vi "Orca Flash Capture Manager.vi"(7 "Calling VI Ref":refnum<vi>) -> ()   [LabVIEW 2016]
uses:
  Orca Flash Capture Manager Controls/Orca Flash Capture Switch Line Scan Modes.ctl
  Orca Flash Capture Manager Controls/Orca Flash Capture Line Scan Settings.ctl
  Orca Flash Capture Manager Controls/Orca Flash Switch Cycles Steps.ctl
  <vilib>/Utility/miscctls.llb/LVPointTypeDef.ctl
  Orca Flash Capture Manager Controls/Orca Flash Capture Notifier Type.ctl
  Orca Flash Capture Manager Controls/Orca Flash Capture Actions.ctl
  <vilib>/vision/Image Controls.llb/IMAQ Image.ctl
  Hardware Configuration/Hardware Configuration Controls/Device Type.ctl
  Orca Flash Capture Manager Controls/Orca Flash Capture Line Scan Filter Settings.ctl
  Tools/Log File/Log File Type Defs/Log File Actions.ctl
  Hardware Configuration/Hardware Configuration Controls/Device Function.ctl
  Device Library/Cameras/Hamamatsu/Orca Flash/Orca Flash Controls/Orca Flash Actions.ctl
  Device Library/Cameras/Hamamatsu/Orca Flash/Orca Flash Controls/Orca Flash Parameters.ctl
  Device Library/Cameras/Hamamatsu/Orca Flash/Orca Flash Controls/Orca Flash Parameter List.ctl
  Device Library/Cameras/Hamamatsu/Orca Flash/Orca Flash Controls/Orca Flash ROI.ctl
  Orca Flash Capture Manager Controls/Orca Flash Capture Cycle Step Count.ctl
  <vilib>/Utility/error.llb/whitespace.ctl
  Device Manager/Common Device Queue/Common Device Controls/Common Device Actions.ctl
  Device Library/SMTP Email Alerts/SMTP Email Alerts Type Defs/SMTP Email Alerts Actions.ctl
  Device Library/DAQmx/AO Single Channel Triggered Ramp/AO SCTR Type Defs/AO SCTR Actions.ctl
  Wide Field Drift Correction/WFDC Controls/WFDC External Sync.ctl
  Wide Field Drift Correction/WFDC Controls/WFDC Cycle Pause.ctl
  Wide Field Drift Correction/WFDC Controls/WFDC Status.ctl
  Device Library/Stages/Stages Controls/Stage Actions.ctl
  Laser Control/Laser Power Control/Laser Power Control Type Defs/Laser Power Ctrl Messenger Actions.ctl
  Device Library/Cameras/Camera Controls/Camera IMAQ Key Info.ctl
  <vilib>/Utility/file.llb/Read Delimited Spreadsheet (DBL).vi
  shell32.dll
panel:
  in  "Main Tab":T1(tab)
  in  "Scan Mode":T2=enum."Cycles Then Steps"
  out "Frame":u32(slide) scale=0.0..20.0
  out "Cycle":sgl(slide) scale=0.0..1.0
  in  "Base Save Path":path
  in  "Capture":bool
  in  "Live Preview":bool
  out "Z Step":sgl(slide) scale=0.0..1.0
  in  "File Name":string="Test Image"
  in  "Preview Exposure Time (s)":dbl=0.1 caption="Frame Rate (Hz)"
  in  "Capture Exposure Time (s)":dbl=0.1 caption="Frame Rate (Hz)"
  in  "No. of Frames":u32=1 min=1
  in  "No. of Cycles":u16=1 min=1
  in  "No. of Z Steps":u16=1 min=1
  in  "Z Step Size (µm)":dbl min=-10.0 max=10.0
  out "Current Cycle":u16
  out "Current Step":u16
  out "Current Frame":u32
  in  "Auto Update Subfolder":bool=TRUE
  in  "Subfolder Name":string="Area"
  in  "Two Color Calibration":bool
  in  "Current Filter":i32(ring) items=["Default"]
  in  "Save As Preset":bool
  in  "Line Scan Active":bool
  in  "Number of Lines":u32=8 min=1 max=200 step=1
  in  "Line Scan Mode":T3
  in  "Line Scanning Presets":u16(ring) items=["04 FPS", "08 FPS Clean", "08 FPS", "40 FPS"]
  in  "Line Scan Settings":T4
  in  "Line Scan Offset Active":bool
  in  "Line Scan Offset (V)":dbl
  in  "Collect Metadata":bool
  in  "Edit Metadata":bool
  in  "Camera Settings":bool
  in  "Quadrants On/Off":bool
  in  "Email Alerts":bool
  in  "Email Address":string
  in  "Auto Laser Off Time (min)":u16=30
  in  "Quit":bool
  # "Live Preview"
  # "Capture"
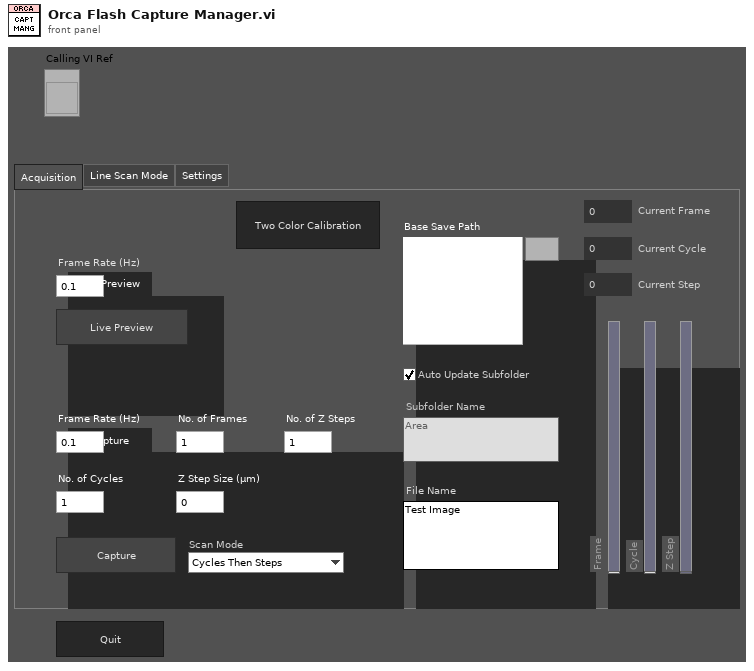
[diagram p1: front panel]
types:
  T1 = enum32{"Acquisition", "Line Scan Mode", "Settings"}
  T2 = typedef "Orca Flash Switch Cycles Steps.ctl" = enum16{"Steps Then Cycles", "Cycles Then Steps"}
  T3 = typedef "Orca Flash Capture Switch Line Scan Modes.ctl" = enum32{"Automatic", "Use Presets", "Manual"}
  T4 = typedef "Orca Flash Capture Line Scan Settings.ctl" = cluster{"Interline Interval":dbl, "Offset (V)":dbl, "Amplitude (V)":dbl, "Samples Per Channel":dbl, "Delay (ms)":dbl}
  T5 = typedef "Log File Actions.ctl" = enum16{"Open File", "Write"}
  T6 = typedef "IMAQ Image.ctl" = refnum<image>
  T7 = cluster{"Image Ref":T6, "Cycle Number":u16, "Camera Running?":bool, "Capture?":bool}
  T8 = typedef "Orca Flash Capture Line Scan Filter Settings.ctl" = cluster{"Filter Name":string, "Offset (V)":dbl}[]
  T9 = enum8{"Enabled", "Disabled", "Disabled and Grayed Out"}
  T10 = typedef "Device Type.ctl" = enum16{"AOTF", "Camera", "Deformable Mirror", "Laser", "Shutter", "Stage", "Waveform", "FPGA", "Email", "Filter Wheel"}
  T11 = typedef "Orca Flash Capture Notifier Type.ctl" = cluster{"Actions":T12, "Running?":bool, "Preview Exposure (s)":dbl, "Capture Exposure (s)":dbl, "Cycles":u16, "Frames":u32, "No. of Z Steps":u16, "Z Step Size (µm)":dbl, "Base Path":path, "Init Z Position (µm)":dbl, "Lasers Lines":string[], "Save Path":path, "Line Scan?":bool, "Line Scan Mode":T3, "Collect Metadata?":bool}
  T12 = typedef "Orca Flash Capture Actions.ctl" = enum16{"Idle", "Live Preview", "Capture", "Check File Name", "Laser On", "Laser Off", "Open Shutters", "Close Shutters", "Set Exposure Time", "Start Acquisition", "Update SubFolder", "Write Metadata", "Setup", "Camera", "Switch", "Step", "Cycle", "External Cycle Sync", "Abort", "Quit"}
  T13 = enum16{"Always On", "Always Off", "Off While Running"}
  T14 = typedef "LVPointTypeDef.ctl" = cluster{"Horizontal":i16, "Vertical":i16}
  T15 = typedef "Image Type" = u32
  T16 = typedef "Device Function.ctl" = enum16{"Primary", "Secondary", "Overview", "Wide Field Drift Correction", "642 nm Excitation", "560 nm Excitation", "940 nm Excitation", "546 nm Excitation", "488 nm Excitation", "405 nm Excitation", "Objective Drift Correction", "4Pi Objective Lock", "Objective XY", "Objective Z", "Sample XY", "Sample Coarse Z", "Sample Z", "4Pi Lower", "4Pi Upper", "Mojo", "Adj Cavity", "Line Scanning", "Alert"}
  T17 = typedef "Orca Flash ROI.ctl" = cluster{"H Offset":i32, "V Offset":i32, "H Width":i32, "V Width":i32}
  T18 = typedef "Orca Flash Parameters.ctl" = cluster{"Value":dbl, "Parameter":T19}
  T19 = typedef "Orca Flash Parameter List.ctl" = u32
  T20 = typedef "Orca Flash Actions.ctl" = enum16{"IDLE", "PREVIEW", "RECORD", "Record Settings", "SETPARAM", "GETPARAM", "SETROI", "GETROI", "PROGRESSIVE MODE", "AREA MODE", "STATUS", "QUIT"}
  T21 = typedef "Orca Flash Capture Cycle Step Count.ctl" = cluster{"Scan Mode":T2, "Current Step":u16, "Current Cycle":u16, "Num of Steps":u16, "Num of Cycles":u16}
  T22 = typedef "WFDC Status.ctl" = enum16{"Idle", "Busy", "DC Active", "Error"}
  T23 = typedef "WFDC External Sync.ctl" = cluster{"Cycle Sync":T24, "Z Offset":dbl, "WFDC Status":T22}
  T24 = typedef "WFDC Cycle Pause.ctl" = enum16{"Pause Requested", "Paused", "Resume Requested", "Resumed"}
  T25 = typedef "SMTP Email Alerts Actions.ctl" = enum16{"Set Recipient", "Send Message", "Quit"}
  T26 = typedef "Stage Actions.ctl" = enum16{"Get Position", "MVR", "MOVE", "HALT", "ONTARGET", "ERROR", "REFERENCE", "INIT", "VELOCITY", "STATUS", "EXIT", "HOME", "ZEROPOS", "NANOPOS", "ANALOG", "QUIT"}
  T27 = typedef "Laser Power Ctrl Messenger Actions.ctl" = enum16{"All Active On", "All Off", "Adjust Power", "Line On/Off", "Get Status"}
  T28 = typedef "AO SCTR Actions.ctl" = enum16{"Stop at Offset", "Update and Run", "Quit"}
  T29 = typedef "Camera IMAQ Key Info.ctl" = cluster{"Frame":u32, "Sensor Height":i32, "Sensor Width":i32, "ROI Height":i32, "ROI Width":i32, "ROI Enable?":bool, "Bit per Pixel":u8}
  T30 = typedef "Common Device Actions.ctl" = enum16{"Specific Action", "Open Front Panel", "Close Front Panel", "Quit", "Quit All"}
  T31 = enum32{"Invalid", "Standard", "Closed", "Hidden", "Minimized", "Maximized"}
  T32 = typedef "whitespace.ctl" = u16
  T33 = typedef "LVRectTypeDef.ctl" = cluster{"Left":i16, "Top":i16, "Right":i16, "Bottom":i16}
  T34 = typedef "LVBoundsTypeDef.ctl" = cluster{"Width":u32, "Height":u32}
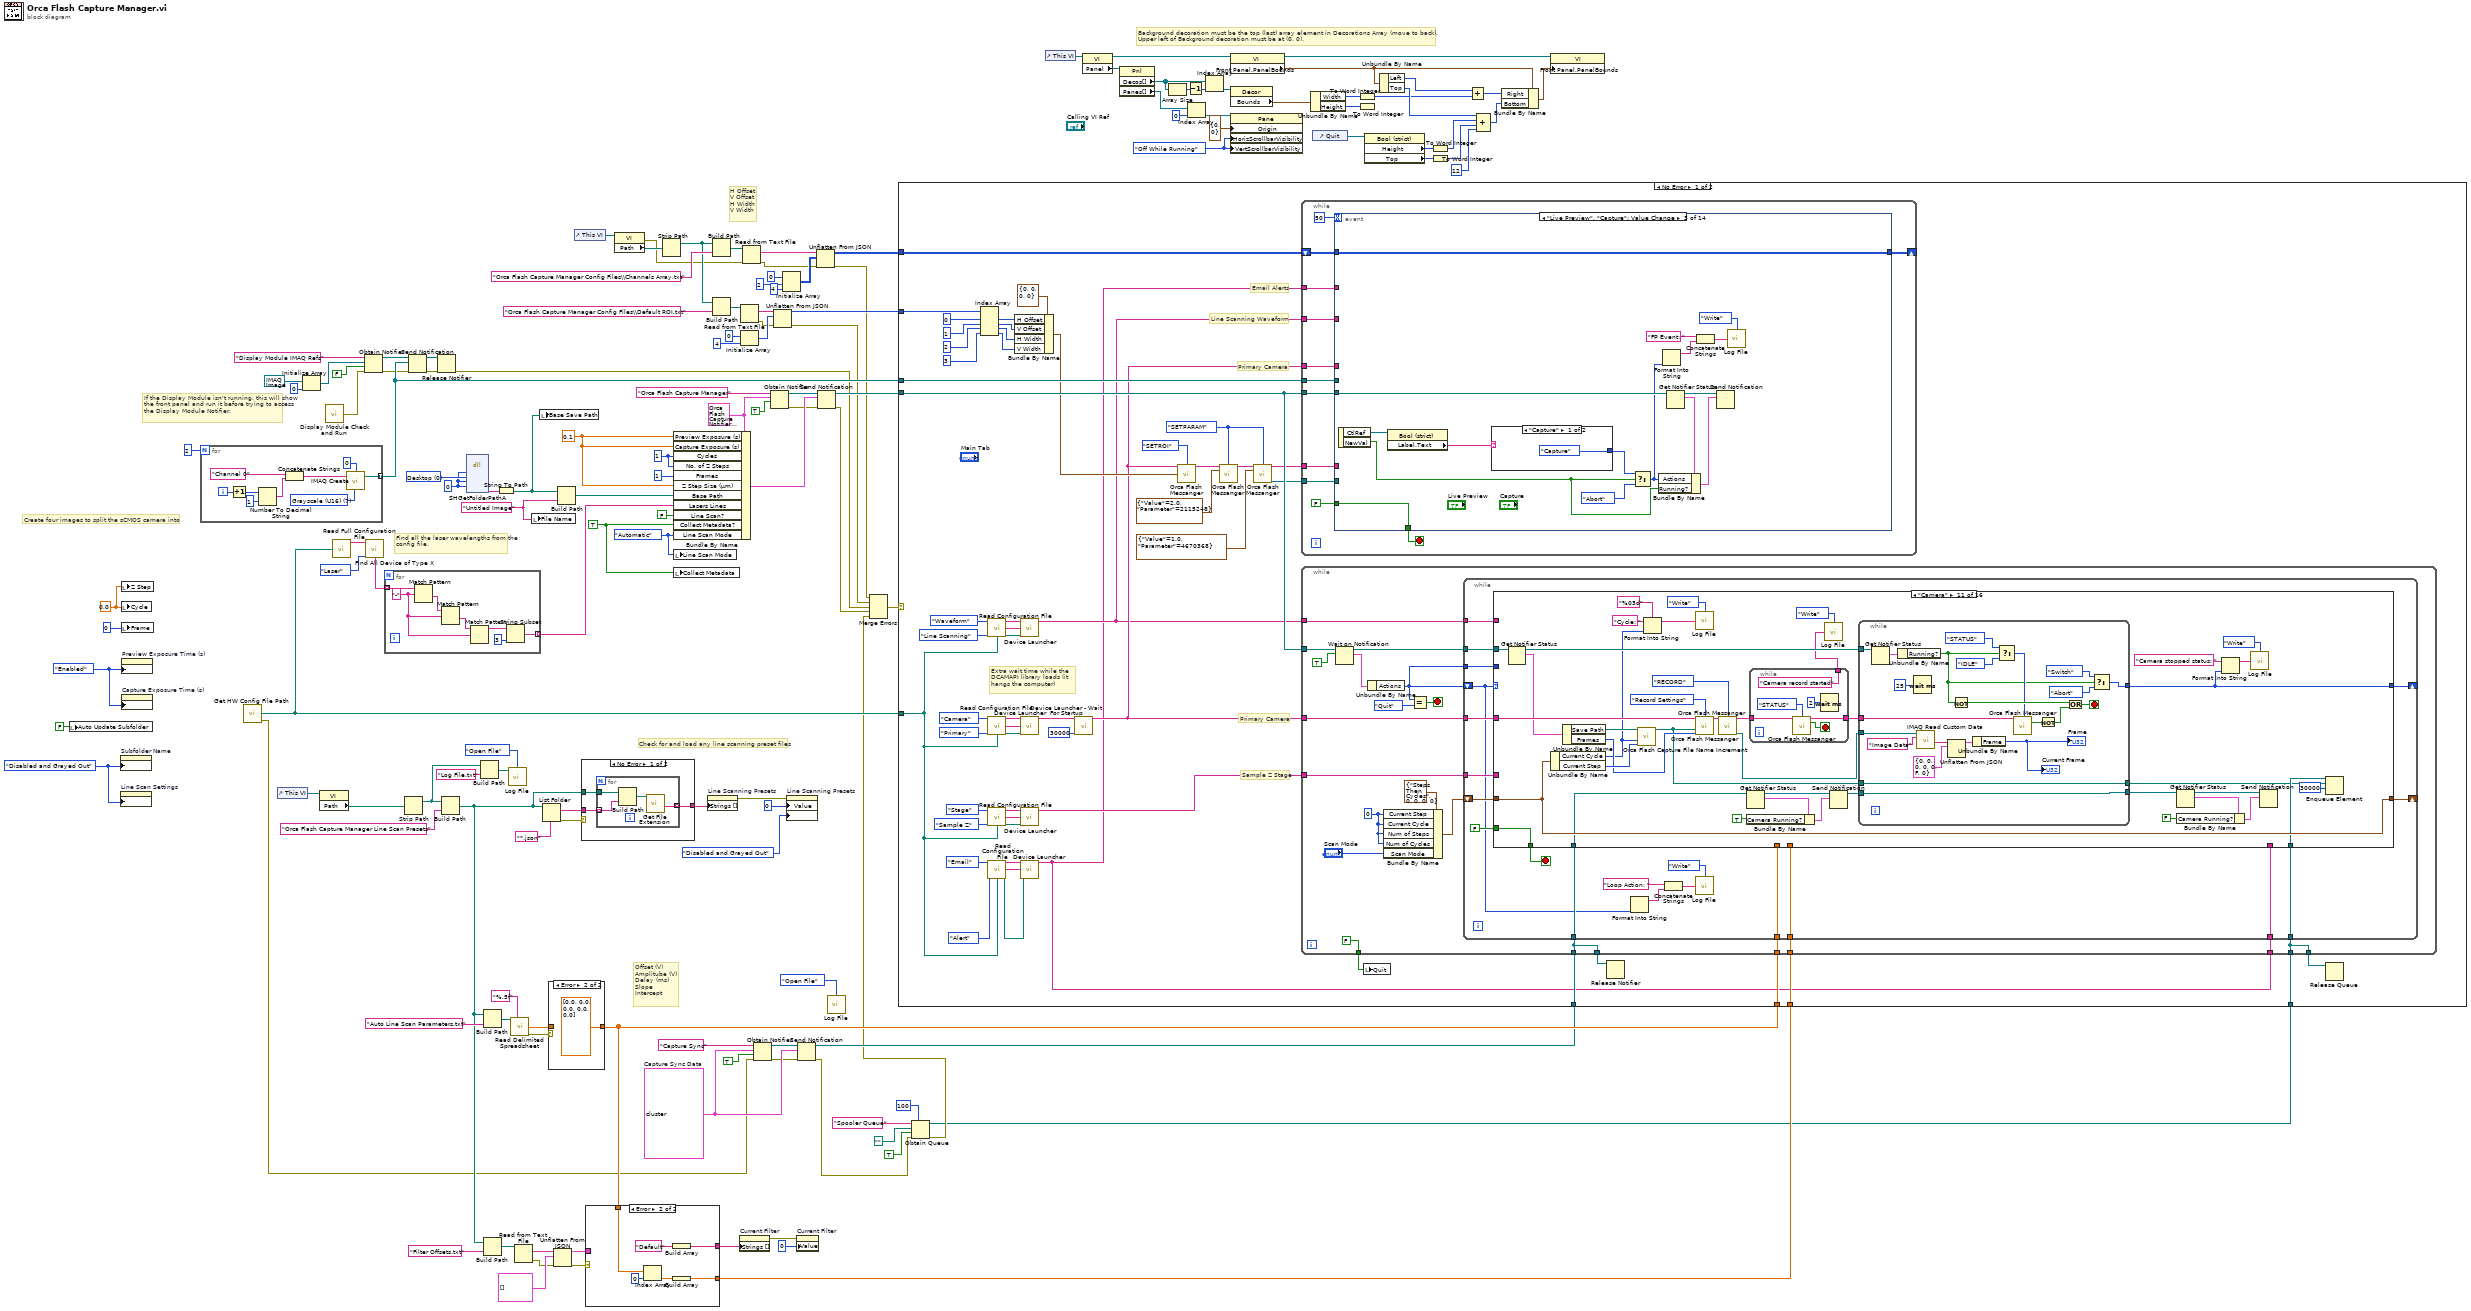
[diagram p0: block diagram]
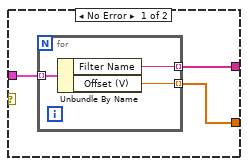
[diagram p2: hidden frame]
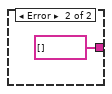
[diagram p4: hidden frame]
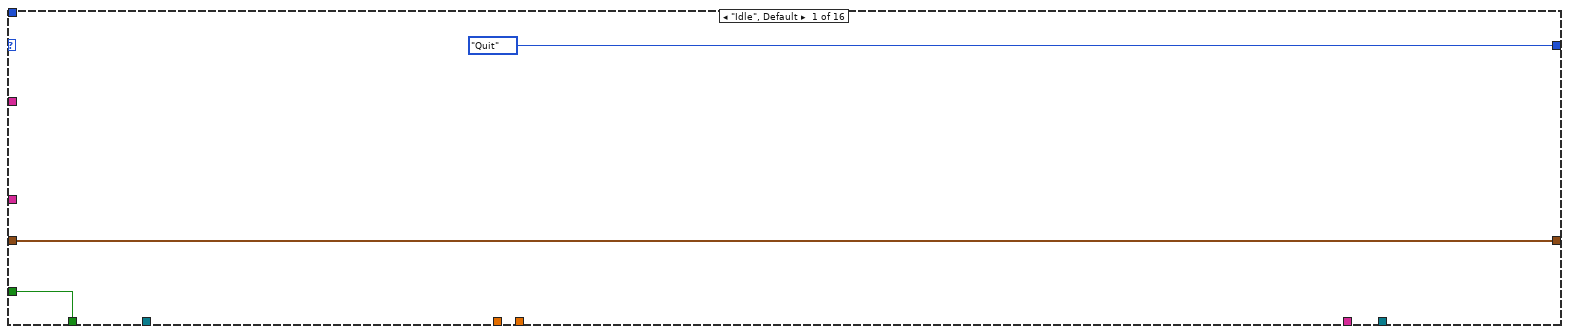
[diagram p5: hidden frame]
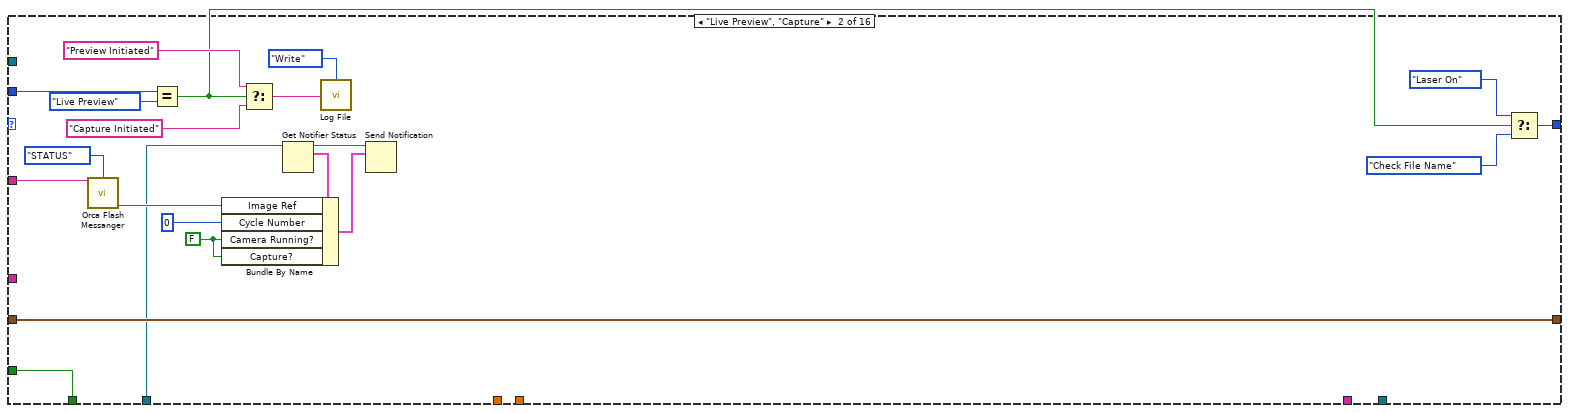
[diagram p6: hidden frame]
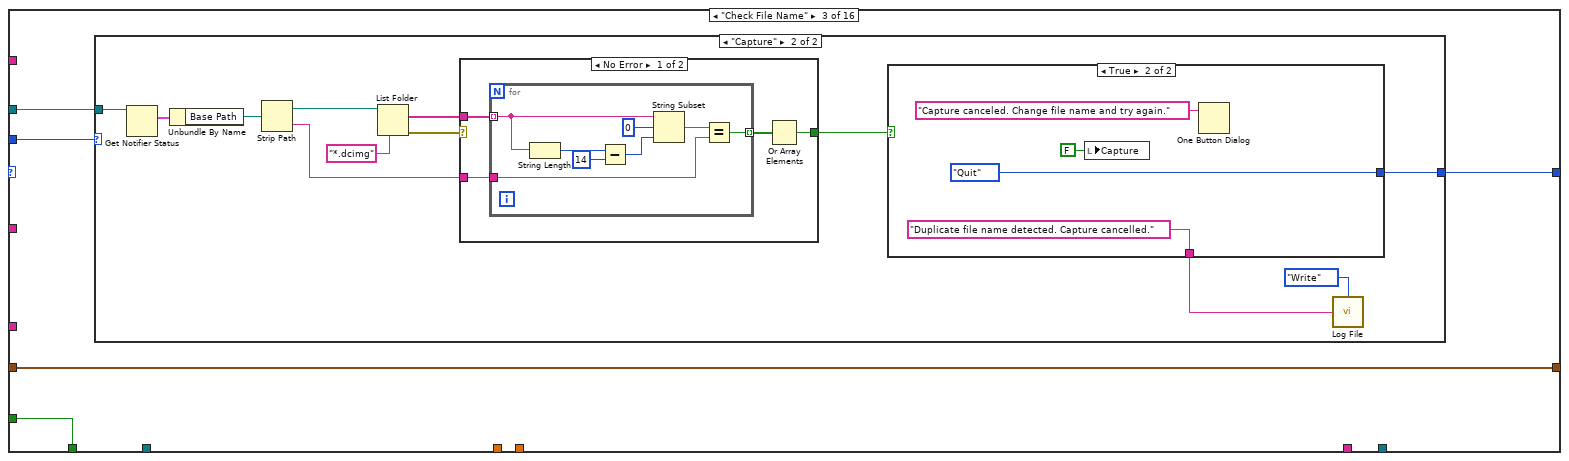
[diagram p7: hidden frame]
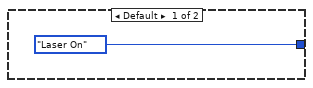
[diagram p8: hidden frame]
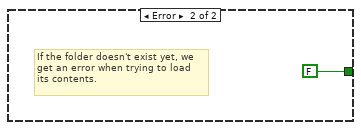
[diagram p9: hidden frame]
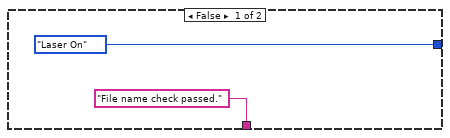
[diagram p10: hidden frame]
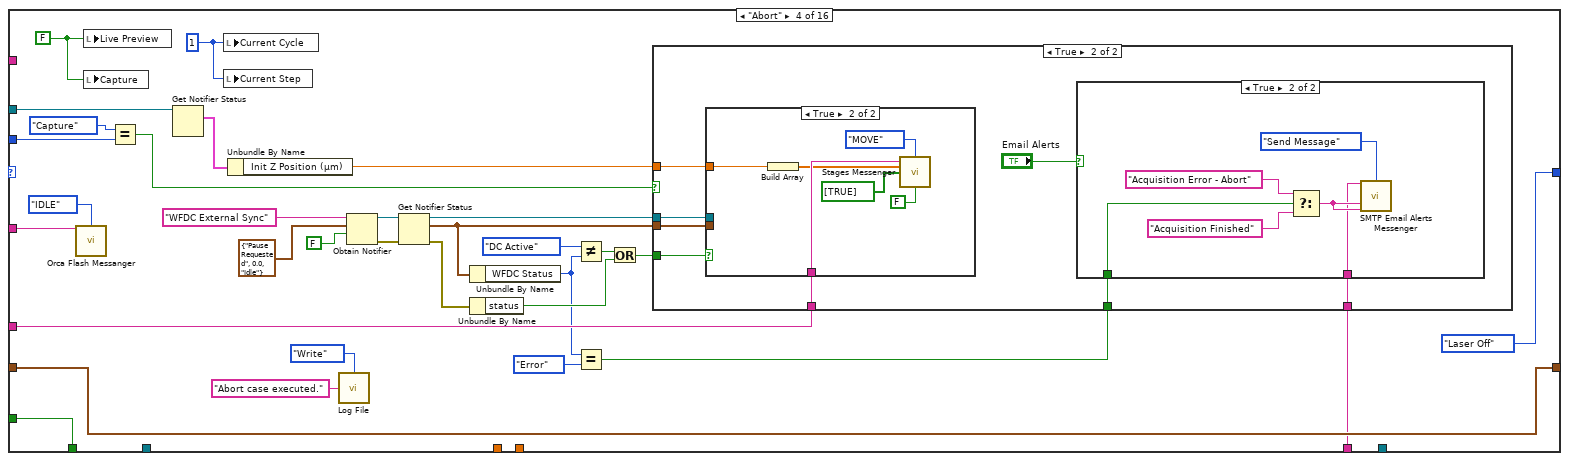
[diagram p11: hidden frame]
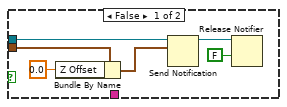
[diagram p14: hidden frame]
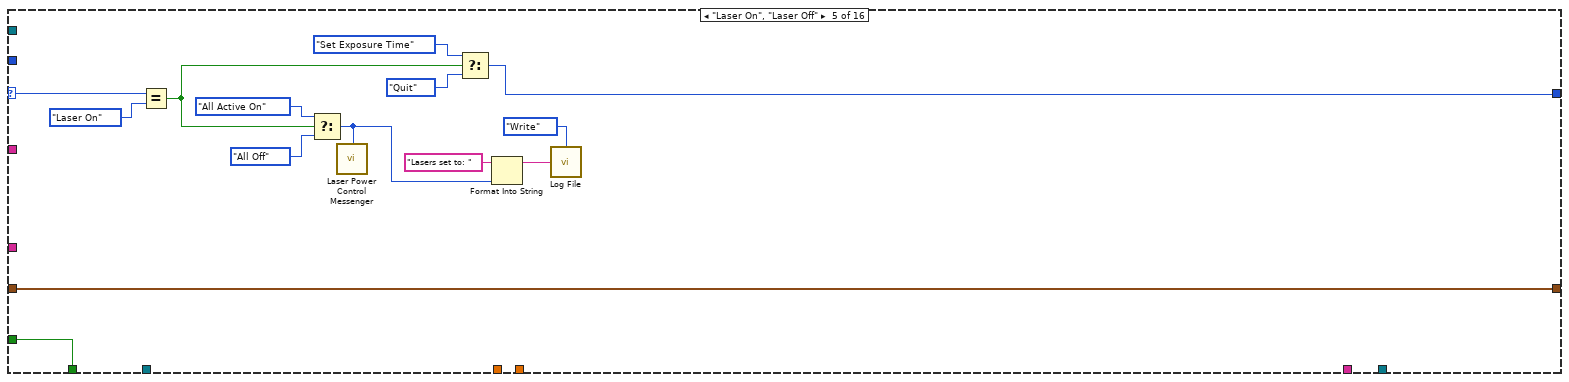
[diagram p15: hidden frame]
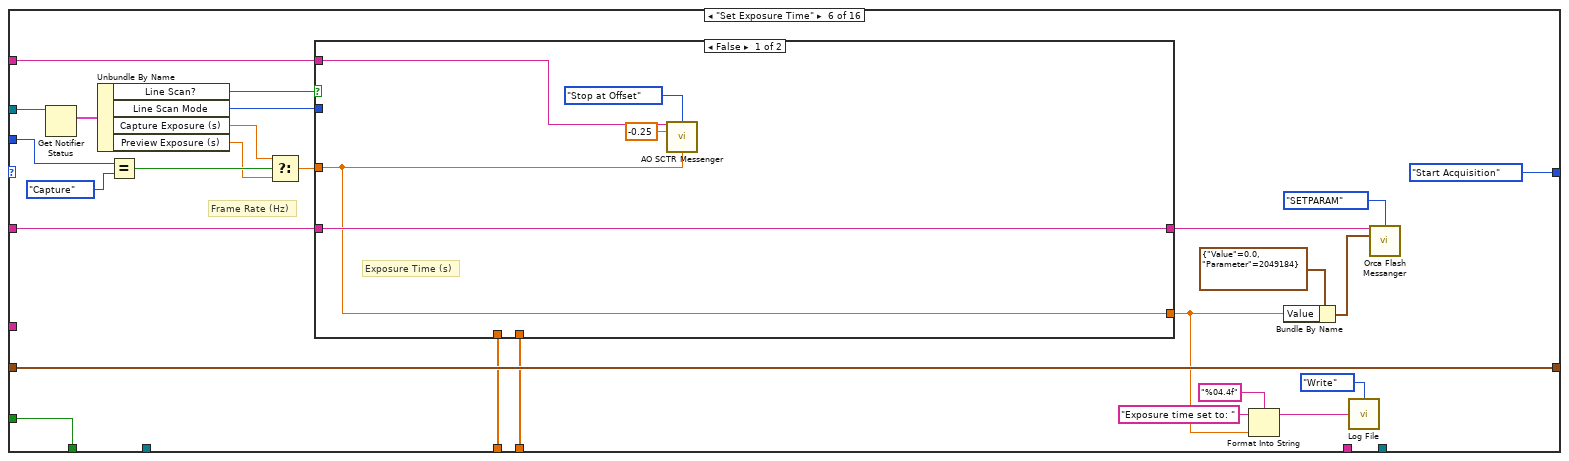
[diagram p16: hidden frame]
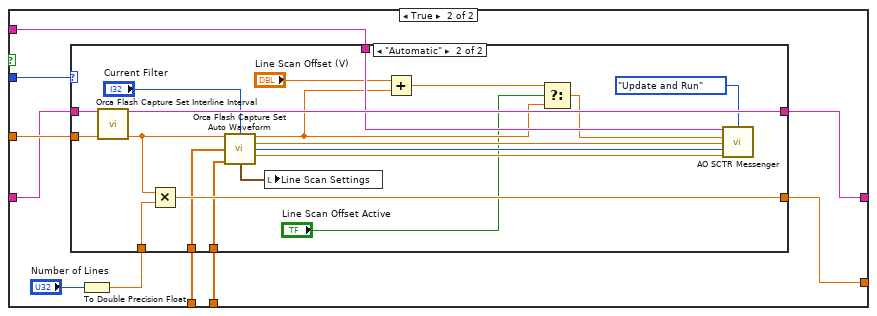
[diagram p17: hidden frame]
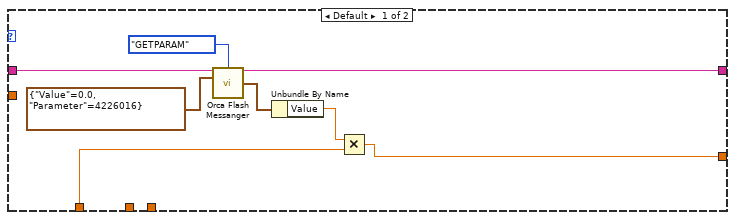
[diagram p18: hidden frame]
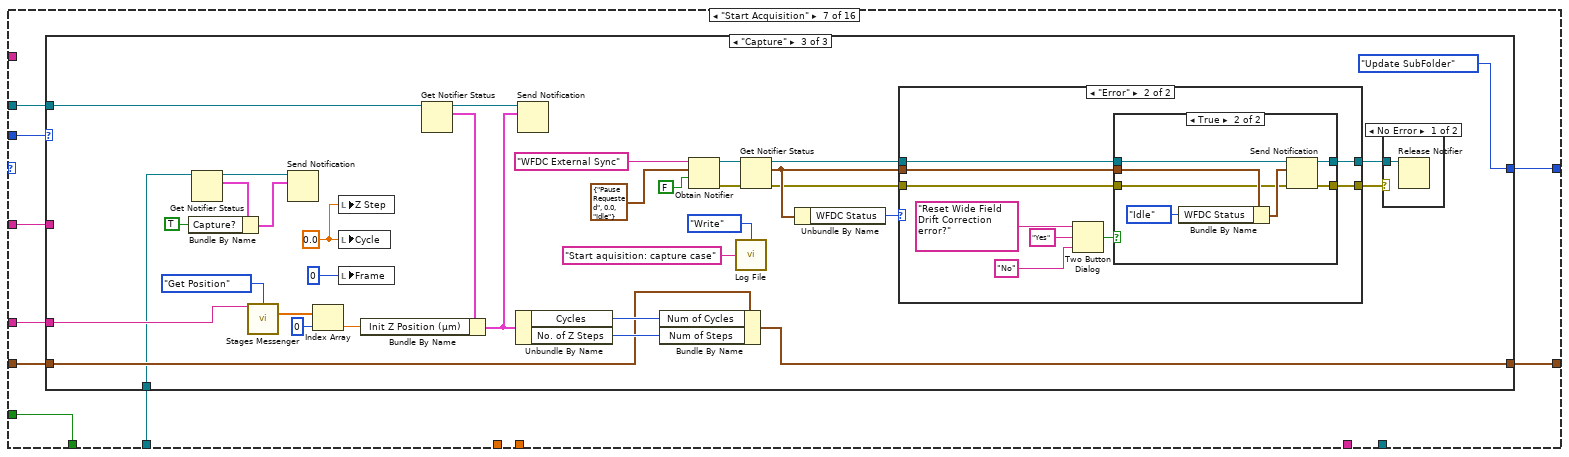
[diagram p19: hidden frame]
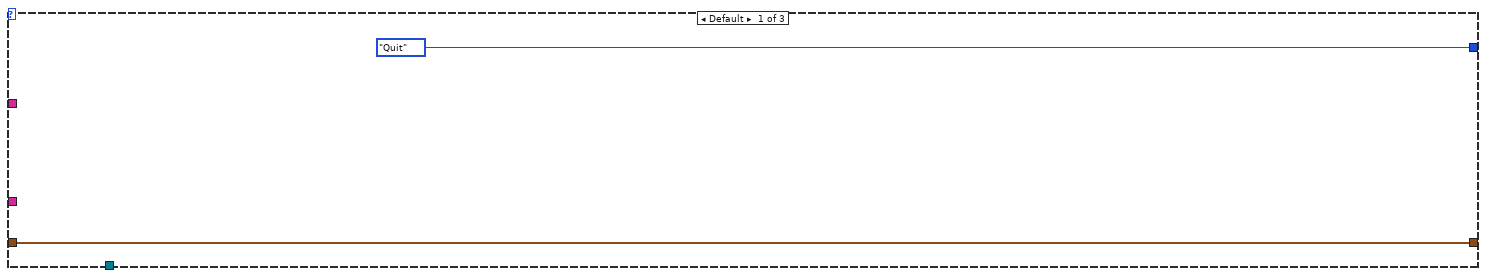
[diagram p20: hidden frame]
diagram:
  w15 = TRUE
  w21 = sgl 0.0 ("Cycle")
  w22 = T7 {"Image Ref"=refnum, "Cycle Number"=0, "Camera Running?"=FALSE, "Capture?"=FALSE}  # Capture Sync Data
  w44 = T9."Enabled" ("Disabled")
  w16 = Orca_Flash_Capture_Switch_Line_Scan_Modes."Automatic" ("Line Scan Mode")
  w45 = T9."Disabled and Grayed Out" ("Disabled")
  w95 = "Untitled Image"
  w98 = 0 items=["Desktop"=0, "Personal Documents"=5, "AppData"=26, "Local AppData"=28, "Common AppData"=35, "Program Files"=38, "Program Files Common"=43, "Common Documents"=46] ("Requested Path")
  w97 = 0 ("HWND")
  w102 = u16 1 ("Cycles")
  w100 = 0.1 ("Preview Exposure (s)")
  w104 = T11 {"Actions"=enum."Live Preview", "Running?"=FALSE, "Preview Exposure (s)"=0.1, "Capture Exposure (s)"=0.1, "Cycles"=1, "Frames"=0, "No. of Z Steps"=0, "Z Step Size (µm)"=0.0, "Base Path"=path "", "Init Z Position (µm)"=0.0, "Lasers Lines"=[], "Save Path"=path "", "Line Scan?"=FALSE, "Line Scan Mode"=enum."Automatic", "Collect Metadata?"=FALSE} ("4Pi Capture Notifier Type")
  w126 = T13."Off While Running" ("Vertical Scrollbar Visibility")
  # "Offset (V)\nAmplitube (V)\nDelay (ms)\nSlope\nIntercept"
  # "Check for and load any line scanning preset files"
  # "Find all the laser wavelengths from the config file."
  # "If the Display Module isn't running, this will show the front panel and run it before trying to access the Display Module Notifier."
  # "H Offset\nV Offset\nH Width\nV Width"
  # "Create four images to split the sCMOS camera into"
  # "Background decoration must be the top (last) array element in Decorations Array (move to back).\nUpper left of Background decoration must be at (0, 0)."
  n1 = local write "Auto Update Subfolder"(FALSE ("Auto Update Subfolder")) -> ()
  n2 = property on="Subfolder Name" class="Str"("DisabledEnum"=w45) -> ()  [unwired: 2 in, 2 out]
  n3 = property on="Line Scan Settings" class="Clust (strict)"("DisabledEnum"=w45) -> ()  [unwired: 2 in, 2 out]
  n4 = local write "Z Step"(w21) -> ()
  n5 = local write "Cycle"(w21) -> ()
  n6 = local write "Frame"(u32 0 ("Frame")) -> ()
  n7 = property on="Preview Exposure Time (s)" class="DigNum (strict)"("DisabledEnum"=w44) -> ()  [unwired: 2 in, 2 out]
  n8 = property on="Capture Exposure Time (s)" class="DigNum (strict)"("DisabledEnum"=w44) -> ()  [unwired: 2 in, 2 out]
  n9 = for {
    N: 2 -> [_]
    tunnel: [w144] -> w108 mode=indexing
    i -> [w152]
    w147 = T15 7 items=["Grayscale (U8)", "Grayscale (I16)", "Grayscale (SGL)", "Complex (CSG)", "RGB (U32)", "HSL (U32)", "RGB (U64)", "Grayscale (U16)"] ("Image Type")
    n10 = Increment(x=w152) -> (x+1=w150:i32)
    n11 = Number To Decimal String(number=w150, width (-)=i16 1) -> (decimal integer string=w148:string)
    n12 = Concatenate Strings("Channel 0" ("name (unnamed)"), w148) -> (w145:string)
    n13 = call "IMAQ Create"("Border Size"=0, "Image Name"=w145, "Image Type"=w147) -> ("New Image"=w144:T6)  [unwired: 2 in, 1 out]
  }
  n14 = call "Get HW Config File Path.vi"() -> ("File Path"=w57:path, "Error"=w19:errorcluster)  [unwired: 14 in]
  n15 = control-ref of="This VI"() -> (w54:refnum<vi>)
  n16 = Initialize Array(T6 refnum ("New Image"), 0 ("dimension size")) -> (w63:T6[])
  n17 = property class="VI"(reference=w54) -> ("Path"=w6:path)  [unwired: 1 in, 2 out]
  n18 = call "Display Module Check and Run.vi"() -> ("Error"=w62:errorcluster)  [unwired: 15 in]
  n19 = call "Read Full Configuration File.vi"("Config File Path"=w57) -> ("Unique Notifier Names"=w59:string[])  [unwired: 11 in, 3 out]
  n20 = Obtain Notifier(name (unnamed)="Display Module IMAQ Refs", notification data type=w63, create if not found? (T)=FALSE, error in (no error)=w62) -> (notifier out=w109:refnum<notifier>, error out=w73:errorcluster)  [unwired: 1 out]
  n21 = call "Find All Device of Type X.vi"("Unique Notifier Names"=w59, "Device Type"=Device_Type."Laser") -> ("All Devices"=w61:string[])  [unwired: 12 in, 1 out]
  n22 = for {
    tunnel: w61 -> [w154] mode=indexing
    tunnel: [w153] -> w58 mode=indexing
    w157 = "-" ("regular expression")
    n23 = Match Pattern(string=w154, regular expression=w157) -> (after substring=w155:string)  [unwired: 1 in, 3 out]
    n24 = Match Pattern(string=w155, regular expression=w157) -> (after substring=w156:string)  [unwired: 1 in, 3 out]
    n25 = Match Pattern(string=w156, regular expression=w157) -> (before substring=w158:string)  [unwired: 1 in, 3 out]
    n26 = String Subset(string=w158, length (rest)=3 ("length (rest)")) -> (substring=w153:string)  [unwired: 1 in]
  }
  n27 = Strip Path(path=w6) -> (stripped path=w4:path)  [unwired: 1 out]
  n28 = Send Notification(notification=w108, notifier=w109, error in (no error)=w73) -> (notifier out=w93:refnum<notifier>, error out=w78:errorcluster)
  n29 = Release Notifier(notifier=w93, error in (no error)=w78) -> (error out=w70:errorcluster)  [unwired: 1 in, 2 out]
  n30 = Build Path(base path=w4, name or relative path="Orca Flash Capture Manager Line Scan Presets") -> (appended path=w38:path)
  n31 = dll-call lib="shell32.dll" fn="SHGetFolderPathA"("HWND"=w97, "nFolder"=w98, "hToken"=w97, "dwFlags"=w97) -> ("pszPath"=w96:string)  [unwired: 9 in, 2 out]
  n32 = Build Path(base path=w4, name or relative path="Log File.txt") -> (appended path=w2:path)
  n33 = Build Path(base path=w38, name or relative path="Auto Line Scan Parameters.txt") -> (appended path=w42:path)
  n34 = Build Path(base path=w38, name or relative path="Filter Offsets.txt") -> (appended path=w36:path)
  n35 = String To Path(string=w96) -> (path=w94:path)
  n36 = call "Log File.vi"("File Path"=w2, "Actions"=Log_File_Actions."Open File") -> ()  [unwired: 14 in]
  n37 = call-poly <vilib>:"Read Delimited Spreadsheet.vi"("file path (dialog if empty)"=w42, "format (%.3f)"="%.5f") -> ("first row"=w39:dbl[], "error out"=w40:errorcluster)  [unwired: 8 in, 4 out]
  n38 = Read from Text File(file (use dialog)=w36) -> (text=w35:string, error out=w33:errorcluster)  [unwired: 3 in, 2 out]
  n39 = local write "File Name"(w95) -> ()
  n40 = local write "Base Save Path"(w94) -> ()
  n41 = List Folder(path=w38, pattern="*.json") -> (filenames=w51:string[], error out=w50:errorcluster)  [unwired: 2 in, 2 out]
  n42 = case shown="Error" w40 {
    tunnel: w39 -> [w160 _]
    tunnel: [w160 dbl[] [0.0, 0.0, 0.0, 0.0, 0.0] ("first row")] -> w30
    frame No Error {
    }
    frame Error {
    }
  }
  n43 = Unflatten From JSON(JSON string=w35, type and defaults=T8 [] ("Line Scan Filter Parameters"), error in (no error)=w33) -> (value=w32:T8, error out=w31:errorcluster)  [unwired: 4 in]
  n44 = Build Path(base path=w94, name or relative path=w95) -> (appended path=w99:path)
  n45 = control-ref of="This VI"() -> (w107:refnum<vi>)
  n46 = case shown="No Error" w50 {
    tunnel: w51 -> [w164 _]
    tunnel: w38 -> [w163 _]
    tunnel: [w162 string[] []] -> w49
    frame No Error {
      n47 = for {
        tunnel: w164 -> [w167] mode=indexing
        tunnel: w163 -> [w168]
        tunnel: [w165] -> w162 mode=indexing
        n48 = Build Path(base path=w168, name or relative path=w167) -> (appended path=w166:path)
        n49 = call <vilib>:"Get File Extension.vi"("file"=w166) -> ("filename without extension"=w165:string)  [unwired: 6 in, 4 out]
      }
    }
    frame Error {
    }
  }
  n50 = case shown="Error" w31 {
    tunnel: w32 -> [w172 _]
    tunnel: w30 -> [_ w180]
    tunnel: [w171 w177] -> w29
    tunnel: [w170 w176] -> w26
    frame No Error {
      n51 = for {
        tunnel: w172 -> [w175] mode=indexing
        tunnel: [w174] -> w171 mode=indexing
        tunnel: [w173] -> w170 mode=indexing
        n52 = Unbundle By Name(w175) -> ("Filter Name"=w174:string, "Offset (V)"=w173:dbl)
      }
    }
    frame Error {
      n53 = Index Array(array=w180, index=0) -> (element=w178:dbl)
      n54 = Build Array("Default") -> (w177:string[])
      n55 = Build Array(w178) -> (w176:dbl[])
    }
  }
  n56 = property class="VI"(reference=w107) -> (error out=w75:errorcluster, "Path"=w106:path)  [unwired: 1 in, 1 out]
  n57 = Strip Path(path=w106) -> (stripped path=w86:path)  [unwired: 1 out]
  n58 = Bundle By Name(cluster=w104, "Preview Exposure (s)"=w100, "Capture Exposure (s)"=w100, "Cycles"=w102, "No. of Z Steps"=w102, "Frames"=u32 1, "Z Step Size (µm)"=w100, "Base Path"=w99, "Lasers Lines"=w58, "Line Scan?"=FALSE, "Collect Metadata?"=w15, "Line Scan Mode"=w16) -> (w103:T11)
  n59 = local write "Line Scan Mode"(w16) -> ()
  n60 = local write "Collect Metadata"(w15) -> ()
  n61 = property on="Line Scanning Presets" class="Ring (strict)"("Strings []"=w49) -> (error out=w48:errorcluster)  [unwired: 2 in, 1 out]
  n62 = Build Path(base path=w86, name or relative path="Orca Flash Capture Manager Config Files\\Channels Array.txt") -> (appended path=w89:path)
  n63 = Build Path(base path=w86, name or relative path="Orca Flash Capture Manager Config Files\\Default ROI.txt") -> (appended path=w84:path)
  n64 = property on="Current Filter" class="Ring (strict)"("Strings []"=w29) -> (error out=w28:errorcluster)  [unwired: 2 in, 1 out]
  n65 = Read from Text File(file (use dialog)=w84) -> (text=w83:string, error out=w76:errorcluster)  [unwired: 3 in, 2 out]
  n66 = Initialize Array(0 ("element"), 4 ("dimension size")) -> (w80:i32[])
  n67 = Read from Text File(file (use dialog)=w89, error in=w75) -> (text=w88:string, error out=w74:errorcluster)  [unwired: 2 in, 2 out]
  n68 = Obtain Notifier(name (unnamed)="Capture Sync", notification data type=w22, create if not found? (T)=TRUE, error in (no error)=w19) -> (notifier out=w23:refnum<notifier>, error out=w18:errorcluster)  [unwired: 1 out]
  n69 = Obtain Notifier(name (unnamed)="Orca Flash Capture Manager", notification data type=w104, create if not found? (T)=TRUE) -> (notifier out=w112:refnum<notifier>, error out=w77:errorcluster)  [unwired: 1 in, 1 out]
  n70 = Unflatten From JSON(JSON string=w83, type and defaults=w80, error in (no error)=w76) -> (value=w79:i32[], error out=w69:errorcluster)  [unwired: 4 in]
  n71 = Initialize Array(0 ("element"), 2 ("dimension size"), 4 ("dimension size")) -> (w90:i32[][])
  n72 = property on="Line Scanning Presets" class="Ring (strict)"(error in=w48, "Value"=u16 0, "DisabledEnum"=T9."Disabled and Grayed Out" ("Disabled")) -> ()  [unwired: 1 in, 2 out]
  n73 = property on="Current Filter" class="Ring (strict)"(error in=w28, "Value"=0) -> ()  [unwired: 1 in, 2 out]
  n74 = Send Notification(notification=w22, notifier=w23, error in (no error)=w18) -> (notifier out=w17:refnum<notifier>, error out=w10:errorcluster)
  n75 = Unflatten From JSON(JSON string=w88, type and defaults=w90, error in (no error)=w74) -> (value=w87:i32[][], error out=w68:errorcluster)  [unwired: 4 in]
  n76 = Send Notification(notification=w103, notifier=w112, error in (no error)=w77) -> (notifier out=w111:refnum<notifier>, error out=w71:errorcluster)
  n77 = call "Log File.vi"("Actions"=Log_File_Actions."Open File") -> ()  [unwired: 15 in]
  n78 = Obtain Queue(max queue size (-1, unlimited)=100, name (unnamed)="Spooler Queue", element data type=path "", create if not found? (T)=TRUE, error in (no error)=w10) -> (queue out=w8:refnum<queue>, error out=w9:errorcluster)  [unwired: 1 out]
  n79 = Merge Errors(w68, w69, w70, w71, w9) -> (w72:errorcluster)
  n80 = case shown="No Error" w72 {
    tunnel: w57 -> [w185 _]
    tunnel: w111 -> [w232 w1316]
    tunnel: w108 -> [w223 w1314]
    tunnel: w87 -> [w222 _]
    tunnel: w79 -> [w213 _]
    tunnel: w30 -> [w194 _]
    tunnel: w26 -> [w193 _]
    tunnel: w17 -> [w192 _]
    tunnel: w8 -> [w183 _]
    frame No Error {
      w218 = Orca_Flash_Actions."SETPARAM" ("Camera Actions")
      # "Email Alerts"
      # "Line Scanning Waveform"
      # "Primary Camera"
      # "Extra wait time while the DCAMAPI library loads (it hangs the computer)"
      # "Sample Z Stage"
      # "Primary Camera"
      n81 = Index Array(array=w213, index #1=0 ("index"), index #2=1 ("index"), index #3=2 ("index"), index #4=3 ("index")) -> (element #1=w208:i32, element #2=w205:i32, element #3=w206:i32, element #4=w207:i32)
      n82 = call "Read Configuration File.vi"("Device Type"=Device_Type."Waveform", "Device Function"=Device_Function."Line Scanning", "Config File Path"=w185) -> ("Unique Notifier Name"=w198:string, "Device Ports/IDs/Channels"=w199:string[], "Device Engine Path"=w196:path)  [unwired: 9 in, 1 out]
      n83 = call "Read Configuration File.vi"("Device Type"=Device_Type."Camera", "Device Function"=Device_Function."Primary", "Config File Path"=w185) -> ("Unique Notifier Name"=w237:string, "Device Ports/IDs/Channels"=w236:string[], "Device Engine Path"=w235:path)  [unwired: 9 in, 1 out]
      n84 = call "Read Configuration File.vi"("Device Type"=Device_Type."Stage", "Device Function"=Device_Function."Sample Z", "Config File Path"=w185) -> ("Unique Notifier Name"=w230:string, "Device Ports/IDs/Channels"=w228:string[], "Device Engine Path"=w227:path)  [unwired: 9 in, 1 out]
      n85 = call "Read Configuration File.vi"("Device Type"=Device_Type."Email", "Device Function"=Device_Function."Alert", "Config File Path"=w185) -> ("Unique Notifier Name"=w188:string, "Device Ports/IDs/Channels"=w187:string[], "Device Engine Path"=w190:path)  [unwired: 9 in, 1 out]
      n86 = Bundle By Name(cluster=T17 {"H Offset"=0, "V Offset"=0, "H Width"=0, "V Width"=0} ("Orca Flash ROI"), "H Offset"=w208, "V Offset"=w205, "H Width"=w206, "V Width"=w207) -> (w204:T17)
      n87 = call "Device Launcher.vi"("Notifier Name"=w198, "Device Ports/IDs/Channels"=w199, "Device Engine Path"=w196) -> ("Notifier Name"=w195:string)  [unwired: 11 in, 1 out]
      n88 = call "Device Launcher.vi"("Notifier Name"=w237, "Device Ports/IDs/Channels"=w236, "Device Engine Path"=w235) -> ("Notifier Name"=w202:string)  [unwired: 11 in, 1 out]
      n89 = call "Device Launcher.vi"("Notifier Name"=w230, "Device Ports/IDs/Channels"=w228, "Device Engine Path"=w227) -> ("Notifier Name"=w225:string)  [unwired: 11 in, 1 out]
      n90 = call "Device Launcher.vi"("Notifier Name"=w188, "Device Ports/IDs/Channels"=w187, "Device Engine Path"=w190) -> ("Notifier Name"=w184:string)  [unwired: 11 in, 1 out]
      n91 = call "Device Launcher - Wait For Startup.vi"("Notifier Name"=w202, "Wait Time (ms)"=30000) -> ("Notifier Name (Dup)"=w201:string)  [unwired: 12 in, 1 out]
      n92 = call "Orca Flash Messanger.vi"("Notifier Name"=w201, "Camera Actions"=Orca_Flash_Actions."SETROI", "sCMOS ROI"=w204) -> ("Notifier Name Dup"=w221:string)  [unwired: 8 in, 4 out]
      n93 = call "Orca Flash Messanger.vi"("Notifier Name"=w221, "Camera Actions"=w218, "sCMOS Parameter"=T18 {"Value"=2.0, "Parameter"=2115248}) -> ("Notifier Name Dup"=w220:string)  [unwired: 8 in, 4 out]
      n94 = call "Orca Flash Messanger.vi"("Notifier Name"=w220, "Camera Actions"=w218, "sCMOS Parameter"=T18 {"Value"=1.0, "Parameter"=4670368}) -> ("Notifier Name Dup"=w219:string, "Image Ref"=w215:T6)  [unwired: 8 in, 3 out]
      n95 = while {
        tunnel: w232 -> [w928]
        tunnel: w219 -> [w927]
        tunnel: w215 -> [w925]
        tunnel: w223 -> [w924]
        shift-right: [w922] -> _
        shift-left: w222 -> [w923]
        tunnel: w201 -> [w921]
        tunnel: w195 -> [w920]
        tunnel: w184 -> [w919]
        stop <- w930 stop-if-true
        n96 = event shown="[2] \"Live Preview\", \"Capture\": Value Change" {
          selector: _ -> [_ _ _ _ _ _ _ _ _ _ _ _ _ _]
          dyn-events: _ -> [_ _ _ _ _ _ _ _ _ _ _ _ _ _]
          timeout: 50 -> [_ _ _ _ _ _ _ _ _ _ _ _ _ _]
          tunnel: [w951 w984 w1066 w1087 w1143 w1168 w1190 w1206 w1230 w1254 w1271 w1287 w1295 w1312] -> w930
          tunnel: FALSE -> [w951 w984 w1066 w1087 w1143 w1168 w1190 w1206 w1230 w1254 w1271 w1287 w1295 _]
          tunnel: w928 -> [w946 w982 w1063 _ _ w1162 w1188 _ w1228 _ _ _ w1290 w1311]
          tunnel: w927 -> [_ w981 _ _ _ _ _ _ _ _ _ _ _ _]
          tunnel: w925 -> [w949 _ _ w1071 _ _ _ _ _ _ _ _ _ _]
          tunnel: w924 -> [w950 _ _ w1077 _ _ _ _ _ _ _ _ _ w1299]
          tunnel: w923 -> [w948 w980 w1057 w1070 w1138 w1145 w1189 w1207 w1229 w1246 w1272 w1286 w1294 w1298]
          tunnel: [w948 w980 w1057 w1069 w1138 w1145 w1189 w1207 w1229 w1246 w1272 w1286 w1294 w1298] -> w922
          tunnel: w921 -> [_ _ _ _ _ w1156 _ _ w1214 _ _ _ _ _]
          tunnel: w920 -> [_ _ _ _ _ w1146 _ _ w1222 _ _ _ _ _]
          tunnel: w919 -> [_ w979 _ _ _ _ _ _ _ _ _ _ _ _]
          event Timeout {
            # "Convert to array and then crop. If you\nextract or mask image the destination\nimage custom data keys are overwritten."
            n97 = event-data() -> ()  [unwired: 1 in, 1 out]
            n98 = call "IMAQ ImageToArray"("Image"=w949) -> ("Image Pixels (U16)"=w947:u16[][])  [unwired: 3 in, 4 out]
            n99 = Get Notifier Status(notifier=w946) -> (current notification=w945:T11, # waiting=w944:i32)  [unwired: 1 in, 3 out]
            n100 = Greater Than 0?(x=w944) -> (x > 0?=w943:bool)
            n101 = for {
              tunnel: w950 -> [w973] mode=indexing
              tunnel: w947 -> [w974]
              tunnel: w948 -> [w971] mode=indexing
              n102 = Index Array(array=w971, index #1=0 ("index"), index #2=2 ("index"), index #3=1 ("index"), index #4=3 ("index")) -> (element #1=w969:i32, element #2=w968:i32, element #3=w964:i32, element #4=w963:i32)
              n103 = Array Subset(array=w974, index (row)=w969, length (row)=w968, index (col)=w964, length (col)=w963) -> (w972:u16[][])
              n104 = call "IMAQ ArrayToImage"("Image Pixels (U16)"=w972, "Image"=w973) -> ()  [unwired: 8 in, 2 out]
            }
            n105 = Unbundle By Name(w945) -> ("Running?"=w934:bool)
            n106 = feedback-in #1(w934) -> ()
            n107 = feedback #1(FALSE) -> (w941:bool)
            n108 = Not(x=w934) -> (.not. x?=w932:bool)
            n109 = Less?(x=w934, y=w941) -> (x < y?=w940:bool)
            n110 = And(x=w940, y=w943) -> (x .and. y?=w937:bool)
            n111 = feedback #2(FALSE) -> (w935:bool)
            n112 = case shown="True" w935 {
              tunnel: [FALSE w957] -> w931
              frame False {
              }
              frame True {
                n113 = feedback #3(u16 0) -> (w961:u16)
                n114 = Multiply(x="Auto Laser Off Time (min)", y=u16 1200) -> (x*y=w954:u16)
                n115 = Increment(x=w961) -> (x+1=w958:u16)
                n116 = Equal?(x=w954, y=w958) -> (x = y?=w957:bool)
                n117 = Select(t=u16 0, s=w957, f=w958) -> (s? t:f=w959:u16)
                n118 = feedback-in #3(w959) -> ()
              }
            }
            n119 = Exclusive Or(1:w931, 2:w937) -> (0:w938:bool)
            n120 = Select(t=w937, s=w938, f=w935) -> (s? t:f=w936:bool)
            n121 = feedback-in #2(w936) -> ()
            n122 = And(x=w931, y=w932) -> (x .and. y?=w933:bool)
            n123 = disable-structure shown="Disabled" {
              disable-tunnel: w933 -> [w952 _]
              frame Disabled {
                # "Turn all laser emission off if capture ends and no activity for X minutes."
                n124 = case shown="True" w952 {
                  frame False {
                  }
                  frame True {
                    n125 = call "All Laser Emission Off.vi"() -> ()  [unwired: 16 in]
                  }
                }
              }
              frame Enabled {
              }
            }
          }
          event "Camera Settings", "Preview Exposure Time (s)", "Capture Exposure Time (s)", "No. of Cycles", "No. of Frames", "No. of Z Steps", "Z Step Size (µm)", "Base Save Path", "File Name", "Email Address": Value Change {
            n126 = event-data() -> ("CtlRef"=w983:refnum<vi>)  [unwired: 1 in]
            n127 = property class="Ctl"(reference=w983) -> ("Label.Text"=w976:string)  [unwired: 1 in, 2 out]
            n128 = Concatenate Strings("FP Event: ", w976) -> (w975:string)
            n129 = case shown="\"Base Save Path\", \"File Name\"" w976 {
              tunnel: w982 -> [_ w988 w996 w1002 w1008 w1022 _ w1038 w1047 _]
              tunnel: w981 -> [_ _ _ _ _ _ w1030 _ _ _]
              tunnel: w979 -> [_ _ _ _ _ _ _ _ _ w1048]
              frame Default {
              }
              frame "No. of Cycles" {
                n130 = Get Notifier Status(notifier=w988) -> (notifier out=w987:refnum<notifier>, current notification=w989:T11)  [unwired: 1 in, 3 out]
                n131 = Bundle By Name(cluster=w989, "Cycles"="No. of Cycles", "Actions"=Orca_Flash_Capture_Actions."Idle") -> (w990:T11)
                n132 = Send Notification(notification=w990, notifier=w987) -> ()  [unwired: 1 in, 2 out]
              }
              frame "No. of Frames" {
                n133 = To Double Precision Float(number="No. of Frames") -> (double precision float=w992:dbl)
                n134 = property on="Frame" class="Slide (strict)"("Scale.Maximum"=w992, "Scale.Minimum"=0.0 ("Scale.Range:Minimum")) -> ()  [unwired: 2 in, 2 out]
                n135 = Get Notifier Status(notifier=w996) -> (notifier out=w995:refnum<notifier>, current notification=w997:T11)  [unwired: 1 in, 3 out]
                n136 = Bundle By Name(cluster=w997, "Frames"="No. of Frames", "Actions"=Orca_Flash_Capture_Actions."Idle") -> (w998:T11)
                n137 = Send Notification(notification=w998, notifier=w995) -> ()  [unwired: 1 in, 2 out]
              }
              frame "No. of Z Steps" {
                n138 = Get Notifier Status(notifier=w1002) -> (notifier out=w1001:refnum<notifier>, current notification=w1003:T11)  [unwired: 1 in, 3 out]
                n139 = Bundle By Name(cluster=w1003, "No. of Z Steps"="No. of Z Steps", "Actions"=Orca_Flash_Capture_Actions."Idle") -> (w1004:T11)
                n140 = Send Notification(notification=w1004, notifier=w1001) -> ()  [unwired: 1 in, 2 out]
              }
              frame "Z Step Size (µm)" {
                n141 = Get Notifier Status(notifier=w1008) -> (notifier out=w1007:refnum<notifier>, current notification=w1009:T11)  [unwired: 1 in, 3 out]
                n142 = Bundle By Name(cluster=w1009, "Z Step Size (µm)"="Z Step Size (µm)", "Actions"=Orca_Flash_Capture_Actions."Idle") -> (w1010:T11)
                n143 = Send Notification(notification=w1010, notifier=w1007) -> ()  [unwired: 1 in, 2 out]
              }
              frame "Base Save Path", "File Name" {
                w1013 = T32 0 items=["both", "start of string", "end of string"] ("location (both)")
                n144 = Path To String(path="Base Save Path") -> (string=w1018:string)
                n145 = Equal?(x="", y=w1018) -> (x = y?=w1016:bool)
                n146 = case shown="True" w1016 {
                  tunnel: [w1025 w1026] -> w1015
                  tunnel: "Base Save Path" -> [w1025 _]
                  frame False {
                  }
                  frame True {
                    w1029 = 0 items=["Desktop"=0, "Personal Documents"=5, "AppData"=26, "Local AppData"=28, "Common AppData"=35, "Program Files"=38, "Program Files Common"=43, "Common Documents"=46] ("Requested Path")
                    w1028 = 0 ("HWND")
                    n147 = dll-call lib="shell32.dll" fn="SHGetFolderPathA"("HWND"=w1028, "nFolder"=w1029, "hToken"=w1028, "dwFlags"=w1028) -> ("pszPath"=w1027:string)  [unwired: 9 in, 2 out]
                    n148 = String To Path(string=w1027) -> (path=w1026:path)
                  }
                }
                n149 = call <vilib>:"Trim Whitespace.vi"("string"="File Name", "location (both)"=w1013) -> ("trimmed string"=w1011:string)
                n150 = Build Path(base path=w1015, name or relative path=w1011) -> (appended path=w1019:path)
                n151 = Get Notifier Status(notifier=w1022) -> (notifier out=w1021:refnum<notifier>, current notification=w1023:T11)  [unwired: 1 in, 3 out]
                n152 = Bundle By Name(cluster=w1023, "Base Path"=w1019, "Actions"=Orca_Flash_Capture_Actions."Idle") -> (w1024:T11)
                n153 = Send Notification(notification=w1024, notifier=w1021) -> ()  [unwired: 1 in, 2 out]
              }
              frame "Camera Settings" {
                n154 = Select(t=Common_Device_Actions."Open Front Panel" ("Common Actions"), s="Camera Settings", f=Common_Device_Actions."Close Front Panel" ("Common Actions")) -> (s? t:f=w1034:T30)
                n155 = call "Common Device Queue Messenger.vi"("Common Action"=w1034, "Notifier Name"=w1030) -> ()  [unwired: 13 in, 1 out]
              }
              frame "Preview Exposure Time (s)" {
                # "Add in a preview stop\nand restart here"
                n156 = Get Notifier Status(notifier=w1038) -> (notifier out=w1041:refnum<notifier>, current notification=w1040:T11)  [unwired: 1 in, 3 out]
                n157 = Bundle By Name(cluster=w1040, "Preview Exposure (s)"="Preview Exposure Time (s)", "Running?"=FALSE ("Abort"), "Actions"=Orca_Flash_Capture_Actions."Idle") -> (w1039:T11)
                n158 = Send Notification(notification=w1039, notifier=w1041) -> ()  [unwired: 1 in, 2 out]
              }
              frame "Capture Exposure Time (s)" {
                n159 = Get Notifier Status(notifier=w1047) -> (notifier out=w1046:refnum<notifier>, current notification=w1045:T11)  [unwired: 1 in, 3 out]
                n160 = Bundle By Name(cluster=w1045, "Capture Exposure (s)"="Capture Exposure Time (s)", "Actions"=Orca_Flash_Capture_Actions."Idle") -> (w1044:T11)
                n161 = Send Notification(notification=w1044, notifier=w1046) -> ()  [unwired: 1 in, 2 out]
              }
              frame "Email Address" {
                n162 = call "SMTP Email Alerts Messenger.vi"("Notifier Name"=w1048, "Actions"=SMTP_Email_Alerts_Actions."Set Recipient", "Recipient"="Email Address") -> ()  [unwired: 13 in]
              }
            }
            n163 = call "Log File.vi"("Actions"=Log_File_Actions."Write", "Message"=w975) -> ()  [unwired: 14 in]
          }
          event "Live Preview", "Capture": Value Change {
            n164 = event-data() -> ("CtlRef"=w1059:refnum<vi>, "NewVal"=w1061:bool)  [unwired: 1 in]
            n165 = property class="Bool (strict)"(reference=w1059) -> ("Label.Text"=w1053:string)  [unwired: 1 in, 2 out]
            n166 = case shown="\"Capture\"" w1053 {
              tunnel: [Orca_Flash_Capture_Actions."Capture" ("y") Orca_Flash_Capture_Actions."Live Preview" ("y")] -> w1058
              frame "Capture" {
              }
              frame "Live Preview", Default {
              }
            }
            n167 = Select(t=w1058, s=w1061, f=Orca_Flash_Capture_Actions."Abort" ("y")) -> (s? t:f=w1052:T12)
            n168 = Format Into String(w1052) -> (resulting string=w1051:string)  [unwired: 3 in, 1 out]
            n169 = Get Notifier Status(notifier=w1063) -> (notifier out=w1064:refnum<notifier>, current notification=w1062:T11)  [unwired: 1 in, 3 out]
            n170 = Bundle By Name(cluster=w1062, "Actions"=w1052, "Running?"=w1061) -> (w1060:T11)
            n171 = Concatenate Strings("FP Event: ", w1051) -> (w1054:string)
            n172 = Send Notification(notification=w1060, notifier=w1064) -> ()  [unwired: 1 in, 2 out]
            n173 = call "Log File.vi"("Actions"=Log_File_Actions."Write", "Message"=w1054) -> ()  [unwired: 14 in]
          }
          event "Quadrants On/Off": Value Change {
            n174 = event-data() -> ("NewVal"=w1083:bool)  [unwired: 1 in]
            n175 = Obtain Notifier(name (unnamed)="Display Module IMAQ Refs", notification data type=T6[] [], create if not found? (T)=FALSE) -> (notifier out=w1076:refnum<notifier>, error out=w1075:errorcluster)  [unwired: 1 in, 1 out]
            n176 = Get Notifier Status(notifier=w1076, error in (no error)=w1075) -> (notifier out=w1074:refnum<notifier>, current notification=w1072:T6[], error out=w1073:errorcluster)  [unwired: 2 out]
            n177 = case shown="False" w1083 {
              tunnel: w1074 -> [w1109 w1124]
              tunnel: w1073 -> [w1108 w1123]
              tunnel: [w1105 w1119] -> w1079
              tunnel: [w1109 w1124] -> w1080
              tunnel: [w1108 w1123] -> w1078
              tunnel: w1077 -> [w1100 w1122]
              tunnel: w1072 -> [w1107 w1121]
              tunnel: w1071 -> [w1101 w1118]
              tunnel: w1070 -> [_ w1117]
              tunnel: [w1088 w1117] -> w1069
              frame False {
                w1099 = 2 ("dimension size")
                n178 = control-ref of="This VI"() -> (w1089:refnum<vi>)
                n179 = Equal?(x=w1107, y=w1101) -> (x = y?=w1104:bool[])
                n180 = property class="VI"(reference=w1089) -> (error out=w1097:errorcluster, "Path"=w1090:path)  [unwired: 1 in, 1 out]
                n181 = for {
                  tunnel: w1104 -> [w1116] mode=indexing
                  tunnel: [w1115] -> w1102
                  i -> [w1115]
                  stop <- w1116 stop-if-true
                }
                n182 = Or Array Elements(Boolean array=w1104) -> (logical OR=w1103:bool)
                n183 = Strip Path(path=w1090) -> (stripped path=w1096:path)  [unwired: 1 out]
                n184 = case shown="True" w1103 {
                  tunnel: w1102 -> [_ w1113]
                  tunnel: w1107 -> [w1110 w1112]
                  tunnel: [w1110 w1111] -> w1106
                  frame False {
                  }
                  frame True {
                    n185 = Delete From Array(array=w1112, length=1, index=w1113) -> (array with subset deleted=w1111:T6[])  [unwired: 1 out]
                  }
                }
                n186 = Build Path(base path=w1096, name or relative path="Orca Flash Capture Manager Config Files\\Channels Array.txt") -> (appended path=w1094:path)
                n187 = Read from Text File(file (use dialog)=w1094, error in=w1097) -> (text=w1095:string, error out=w1098:errorcluster)  [unwired: 2 in, 2 out]
                n188 = Initialize Array(0 ("element"), w1099, w1099) -> (w1093:i32[][])
                n189 = Build Array (concatenate)(w1106, w1100) -> (w1105:T6[])
                n190 = Unflatten From JSON(JSON string=w1095, type and defaults=w1093, error in (no error)=w1098) -> (value=w1088:i32[][])  [unwired: 4 in, 1 out]
              }
              frame True {
                n191 = for {
                  tunnel: w1122 -> [w1127] mode=indexing
                  shift-right: [w1125] -> w1120
                  shift-left: w1121 -> [w1126]
                  n192 = Equal?(x=w1126, y=w1127) -> (x = y?=w1130:bool[])
                  n193 = for {
                    tunnel: w1130 -> [w1137] mode=indexing
                    tunnel: [w1136] -> w1128
                    i -> [w1136]
                    stop <- w1137 stop-if-true
                  }
                  n194 = Or Array Elements(Boolean array=w1130) -> (logical OR=w1129:bool)
                  n195 = case shown="True" w1129 {
                    tunnel: w1128 -> [_ w1134]
                    tunnel: w1126 -> [w1131 w1133]
                    tunnel: [w1131 w1132] -> w1125
                    frame False {
                    }
                    frame True {
                      n196 = Delete From Array(array=w1133, length=1, index=w1134) -> (array with subset deleted=w1132:T6[])  [unwired: 1 out]
                    }
                  }
                }
                n197 = Build Array (concatenate)(w1120, w1118) -> (w1119:T6[])
              }
            }
            n198 = Send Notification(notification=w1079, notifier=w1080, error in (no error)=w1078) -> (notifier out=w1082:refnum<notifier>, error out=w1081:errorcluster)
            n199 = Release Notifier(notifier=w1082, error in (no error)=w1081) -> ()  [unwired: 1 in, 3 out]
          }
          event "Auto Update Subfolder": Value Change {
            n200 = event-data() -> ("NewVal"=w1142:bool)  [unwired: 1 in]
            n201 = Select(t=T9."Enabled" ("Disabled"), s=w1142, f=T9."Disabled and Grayed Out") -> (s? t:f=w1139:T9)
            n202 = property on="Subfolder Name" class="Str"("DisabledEnum"=w1139) -> ()  [unwired: 2 in, 2 out]
          }
          event "Line Scan Active": Value Change {
            n203 = event-data() -> ("NewVal"=w1144:bool)  [unwired: 1 in]
            n204 = Select(t="Frame Rate (Hz)", s=w1144, f="Exposure Time (s)") -> (s? t:f=w1165:string)
            n205 = Select(t=4.0, s=w1144, f=0.1) -> (s? t:f=w1158:dbl)
            n206 = Select(t=-1.0 ("f"), s=w1144, f=0.0) -> (s? t:f=w1149:dbl)
            n207 = Select(t=AO_SCTR_Actions."Update and Run" ("Actions"), s=w1144, f=AO_SCTR_Actions."Stop at Offset" ("Actions")) -> (s? t:f=w1150:T28)
            n208 = property on="Capture Exposure Time (s)" class="DigNum (strict)"("Caption.Text"=w1165, "Value"=w1158) -> ()  [unwired: 2 in, 2 out]
            n209 = property on="Preview Exposure Time (s)" class="DigNum (strict)"("Caption.Text"=w1165, "Value"=w1158) -> ()  [unwired: 2 in, 2 out]
            n210 = call "AO SCTR Messenger.vi"("Notifier Name"=w1146, "Actions"=w1150, "Offset (V)"=w1149) -> ()  [unwired: 12 in, 1 out]
            n211 = case shown="False" w1144 {
              frame False {
                w1169 = T9."Enabled" ("Disabled")
                n212 = property on="Preview Exposure Time (s)" class="DigNum (strict)"("DisabledEnum"=w1169) -> ()  [unwired: 2 in, 2 out]
                n213 = property on="Capture Exposure Time (s)" class="DigNum (strict)"("DisabledEnum"=w1169) -> ()  [unwired: 2 in, 2 out]
              }
              frame True {
              }
            }
            n214 = Get Notifier Status(notifier=w1162) -> (notifier out=w1161:refnum<notifier>, current notification=w1160:T11)  [unwired: 1 in, 3 out]
            n215 = Bundle By Name(cluster=w1160, "Line Scan?"=w1144, "Actions"=Orca_Flash_Capture_Actions."Idle", "Preview Exposure (s)"=w1158, "Capture Exposure (s)"=w1158) -> (w1157:T11)
            n216 = Select(t=Orca_Flash_Actions."PROGRESSIVE MODE" ("Camera Actions"), s=w1144, f=Orca_Flash_Actions."AREA MODE" ("Camera Actions")) -> (s? t:f=w1153:T20)
            n217 = call "Orca Flash Messanger.vi"("Notifier Name"=w1156, "Camera Actions"=w1153) -> ()  [unwired: 9 in, 5 out]
            n218 = Send Notification(notification=w1157, notifier=w1161) -> ()  [unwired: 1 in, 2 out]
          }
          event Value Change {
            n219 = event-data() -> ("NewVal"=w1179:T3)  [unwired: 1 in]
            n220 = Get Notifier Status(notifier=w1188) -> (notifier out=w1187:refnum<notifier>, current notification=w1186:T11)  [unwired: 1 in, 3 out]
            n221 = Bundle By Name(cluster=w1186, "Actions"=Orca_Flash_Capture_Actions."Idle", "Line Scan Mode"=w1179) -> (w1185:T11)
            n222 = Send Notification(notification=w1185, notifier=w1187) -> ()  [unwired: 1 in, 2 out]
            n223 = Equal?(x=w1179, y=Orca_Flash_Capture_Switch_Line_Scan_Modes."Use Presets") -> (x = y?=w1171:bool)
            n224 = Not Equal?(x=w1179, y=Orca_Flash_Capture_Switch_Line_Scan_Modes."Automatic") -> (x != y?=w1173:bool)
            n225 = Select(t=T9."Enabled" ("Disabled"), s=w1171, f=T9."Enabled" ("Disabled")) -> (s? t:f=w1181:T9)
            n226 = property on="Line Scanning Presets" class="Ring (strict)"("DisabledEnum"=w1181) -> ()  [unwired: 2 in, 2 out]
            n227 = case shown="True" w1171 {
              frame False {
              }
              frame True {
                n228 = property on="Line Scanning Presets" class="Ring (strict)"() -> ("Value"=w1191:u16)  [unwired: 2 in, 2 out]
                n229 = property on="Line Scanning Presets" class="Ring (strict)"("Val(Sgnl)"=w1191) -> ()  [unwired: 2 in, 2 out]
              }
            }
            n230 = Select(t=T9."Disabled and Grayed Out" ("Disabled"), s=w1173, f=T9."Enabled" ("Disabled")) -> (s? t:f=w1172:T9)
            n231 = Select(t=T9."Enabled" ("Disabled"), s=w1173, f=T9."Enabled" ("Disabled")) -> (s? t:f=w1176:T9)
            n232 = property on="Preview Exposure Time (s)" class="DigNum (strict)"("DisabledEnum"=w1172) -> ()  [unwired: 2 in, 2 out]
            n233 = property on="Capture Exposure Time (s)" class="DigNum (strict)"("DisabledEnum"=w1172) -> ()  [unwired: 2 in, 2 out]
            n234 = property on="Save As Preset" class="Bool"("DisabledEnum"=w1176) -> ()  [unwired: 2 in, 2 out]
            n235 = property on="Line Scan Settings" class="Clust (strict)"("DisabledEnum"=w1176) -> ()  [unwired: 2 in, 2 out]
          }
          event "Line Scanning Presets": Value Change {
            n236 = event-data() -> ("CtlRef"=w1201:refnum<vi>)  [unwired: 1 in]
            n237 = control-ref of="This VI"() -> (w1205:refnum<vi>)
            n238 = property class="Ring (strict)"(reference=w1201) -> ("RingText.Text"=w1199:string)  [unwired: 1 in, 2 out]
            n239 = property class="VI"(reference=w1205) -> ("Path"=w1204:path)  [unwired: 1 in, 2 out]
            n240 = Strip Path(path=w1204) -> (stripped path=w1203:path)  [unwired: 1 out]
            n241 = Concatenate Strings(w1199, ".json" ("string")) -> (w1197:string)
            n242 = Build Path(base path=w1203, name or relative path="Orca Flash Capture Manager Line Scan Presets") -> (appended path=w1200:path)
            n243 = Build Path(base path=w1200, name or relative path=w1197) -> (appended path=w1196:path)
            n244 = Read from Text File(file (use dialog)=w1196) -> (text=w1195:string, error out=w1193:errorcluster)  [unwired: 3 in, 2 out]
            n245 = Unflatten From JSON(JSON string=w1195, type and defaults=T4 {"Interline Interval"=0.0, "Offset (V)"=0.0, "Amplitude (V)"=0.0, "Samples Per Channel"=0.0, "Delay (ms)"=0.0} ("Line Scan Settings"), error in (no error)=w1193) -> (value=w1192:T4)  [unwired: 4 in, 1 out]
            n246 = property on="Line Scan Settings" class="Clust (strict)"("Val(Sgnl)"=w1192) -> ()  [unwired: 2 in, 2 out]
          }
          event Value Change {
            # "If you try and set the ILI while the camera is in area mode it gives an error"
            n247 = event-data() -> ("NewVal"=w1223:T4)  [unwired: 1 in]
            n248 = Get Notifier Status(notifier=w1228) -> (current notification=w1227:T11)  [unwired: 1 in, 4 out]
            n249 = Unbundle By Name(w1223) -> ("Offset (V)"=w1217:dbl, "Amplitude (V)"=w1221:dbl, "Samples Per Channel"=w1220:dbl, "Delay (ms)"=w1219:dbl, "Interline Interval"=w1212:dbl)
            n250 = Unbundle By Name(w1227) -> ("Line Scan?"=w1210:bool)
            n251 = To Long Integer(number=w1220) -> (32bit integer=w1218:i32)
            n252 = feedback-in #4(w1212) -> ()
            n253 = feedback #4(0.0) -> (w1211:dbl)
            n254 = Select(t=w1217, s=w1210, f=0.0) -> (s? t:f=w1215:dbl)
            n255 = Not Equal?(x=w1212, y=w1211) -> (x != y?=w1208:bool)
            n256 = Select(t=AO_SCTR_Actions."Update and Run" ("Actions"), s=w1210, f=AO_SCTR_Actions."Stop at Offset" ("Actions")) -> (s? t:f=w1224:T28)
            n257 = call "AO SCTR Messenger.vi"("Notifier Name"=w1222, "Actions"=w1224, "Offset (V)"=w1215, "Amplitude (V)"=w1221, "Samples Per Channel"=w1218, "Start Delay (ms)"=w1219) -> ()  [unwired: 9 in, 1 out]
            n258 = And(x=w1210, y=w1208) -> (x .and. y?=w1209:bool)
            n259 = case shown="True" w1209 {
              tunnel: w1214 -> [_ w1233]
              tunnel: w1212 -> [_ w1232]
              frame False {
              }
              frame True {
                n260 = Bundle By Name(cluster=T18 {"Value"=0.0, "Parameter"=4226016} ("sCMOS Parameter"), "Value"=w1232) -> (w1236:T18)
                n261 = call "Orca Flash Messanger.vi"("Notifier Name"=w1233, "Camera Actions"=Orca_Flash_Actions."SETPARAM", "sCMOS Parameter"=w1236) -> ("sCMOS Parameter"=w1237:T18)  [unwired: 8 in, 4 out]
                n262 = Unbundle By Name(w1237) -> ("Value"=w1231:dbl)
                n263 = property on="Interline Interval" class="DigNum (strict)"("Value"=w1231) -> ()  [unwired: 2 in, 2 out]
              }
            }
          }
          event "Save As Preset": Value Change {
            n264 = event-data() -> ()  [unwired: 1 in, 6 out]
            n265 = control-ref of="This VI"() -> (w1250:refnum<vi>)
            n266 = property class="VI"(reference=w1250) -> ("Path"=w1249:path)  [unwired: 1 in, 2 out]
            n267 = Strip Path(path=w1249) -> (stripped path=w1248:path)  [unwired: 1 out]
            n268 = Build Path(base path=w1248, name or relative path="Orca Flash Capture Manager Line Scan Presets") -> (appended path=w1239:path)
            n269 = call "File Dialog"("start path"=w1239, "prompt"="Save Preset File", "pattern (all files)"="*.json", "pattern label"="JSON") -> ("selected path"=w1244:path, "error out"=w1245:errorcluster)  [unwired: 8 in, 2 out]
            n270 = case shown="No Error" w1245 {
              selector: w1245 -> [_ w1270]
              tunnel: w1244 -> [w1269 _]
              tunnel: [w1263 w1270] -> w1238
              frame No Error {
                n271 = local read "Line Scan Settings"() -> (w1268:T4)
                n272 = Flatten To JSON(anything=w1268) -> (JSON string=w1267:string, 11:w1266:errorcluster)  [unwired: 2 in]
                n273 = Write to Text File(file (use dialog)=w1269, text=w1267, error in=w1266) -> (refnum out=w1265:refnum<file>, error out=w1264:errorcluster)  [unwired: 1 in, 1 out]
                n274 = Close File(refnum=w1265, error in=w1264) -> (error out=w1263:errorcluster)  [unwired: 1 out]
              }
              frame Error {
              }
            }
            n275 = List Folder(path=w1239, pattern="*.json", error in=w1238) -> (filenames=w1242:string[], error out=w1241:errorcluster)  [unwired: 1 in, 2 out]
            n276 = case shown="No Error" w1241 {
              tunnel: w1242 -> [w1257 _]
              tunnel: w1239 -> [w1256 _]
              tunnel: [w1255 string[] []] -> w1240
              frame No Error {
                n277 = for {
                  tunnel: w1257 -> [w1260] mode=indexing
                  tunnel: w1256 -> [w1261]
                  tunnel: [w1258] -> w1255 mode=indexing
                  n278 = Build Path(base path=w1261, name or relative path=w1260) -> (appended path=w1259:path)
                  n279 = call <vilib>:"Get File Extension.vi"("file"=w1259) -> ("filename without extension"=w1258:string)  [unwired: 6 in, 4 out]
                }
              }
              frame Error {
              }
            }
            n280 = property on="Line Scanning Presets" class="Ring (strict)"("Strings []"=w1240) -> ()  [unwired: 2 in, 2 out]
          }
          event "Edit Metadata": Value Change {
            n281 = event-data() -> ()  [unwired: 1 in, 1 out]
            n282 = call "Edit Sample Metadata.vi"() -> ()  [unwired: 14 in, 2 out]
          }
          event "Two Color Calibration": Value Change {
            n283 = event-data() -> ()  [unwired: 1 in, 6 out]
            n284 = control-ref of="This VI"() -> (w1285:refnum<vi>)
            n285 = property class="VI"(reference=w1285) -> ("Path"=w1284:path)  [unwired: 1 in, 2 out]
            n286 = Strip Path(path=w1284) -> (stripped path=w1283:path)  [unwired: 1 out]
            n287 = Strip Path(path=w1283) -> (stripped path=w1282:path)  [unwired: 1 out]
            n288 = Build Path(base path=w1282, name or relative path="Two Color Calibration\\Two Color Calibration.vi") -> (appended path=w1280:path)
            n289 = Open VI Reference(vi path=w1280) -> (vi reference=w1276:refnum<vi>)  [unwired: 5 in, 1 out]
            n290 = invoke class="VI" method="FP.Open"(reference=w1276, "Activate"=TRUE ("Activate?"), "State"=T31."Standard") -> (reference out=w1275:refnum<vi>)  [unwired: 2 in, 4 out]
            n291 = invoke class="VI" method="Run VI"(reference=w1275, "Wait until done"=FALSE ("Wait Until Done")) -> (reference out=w1278:refnum<vi>)  [unwired: 3 in, 4 out]
            n292 = invoke class="VI" method="FP.Center"(reference=w1278) -> (reference out=w1277:refnum<vi>)  [unwired: 2 in, 2 out]
            n293 = Close Reference(reference=w1277) -> ()  [unwired: 1 in, 1 out]
          }
          event "Collect Metadata": Value Change {
            n294 = event-data() -> ("NewVal"=w1288:bool)  [unwired: 1 in]
            n295 = Get Notifier Status(notifier=w1290) -> (notifier out=w1293:refnum<notifier>, current notification=w1292:T11)  [unwired: 1 in, 3 out]
            n296 = Bundle By Name(cluster=w1292, "Actions"=Orca_Flash_Capture_Actions."Idle", "Collect Metadata?"=w1288) -> (w1291:T11)
            n297 = Send Notification(notification=w1291, notifier=w1293) -> ()  [unwired: 1 in, 2 out]
          }
          event "Quit": Value Change {
            n298 = event-data() -> ("NewVal"=w1312:bool)  [unwired: 1 in]
            n299 = Get Notifier Status(notifier=w1311) -> (notifier out=w1310:refnum<notifier>, current notification=w1309:T11)  [unwired: 1 in, 3 out]
            n300 = Bundle By Name(cluster=w1309, "Running?"=FALSE ("Abort"), "Actions"=Orca_Flash_Capture_Actions."Quit") -> (w1303:T11)
            n301 = Send Notification(notification=w1303, notifier=w1310) -> (notifier out=w1307:refnum<notifier>)  [unwired: 1 in, 1 out]
            n302 = Wait on Notification(notifier=w1307, ignore previous (F)=TRUE, timeout in ms (-1)=500) -> (notifier out=w1304:refnum<notifier>)  [unwired: 1 in, 3 out]
            n303 = Send Notification(notification=w1303, notifier=w1304) -> (notifier out=w1301:refnum<notifier>)  [unwired: 1 in, 1 out]
            n304 = call "Log File.vi"("Actions"=Log_File_Actions."Write", "Message"="FP Event: Quit") -> ()  [unwired: 14 in]
            n305 = Release Notifier(notifier=w1301, force destroy? (F)=TRUE) -> ()  [unwired: 1 in, 3 out]
            n306 = for {
              tunnel: w1299 -> [w1313] mode=indexing
              n307 = call "IMAQ Dispose"("Image"=w1313) -> ()  [unwired: 5 in, 1 out]
            }
          }
        }
      }
      n308 = while {
        tunnel: w232 -> [w257]
        tunnel: w201 -> [w251]
        tunnel: [FALSE] -> w231
        tunnel: w225 -> [w248]
        tunnel: w195 -> [w246]
        tunnel: w194 -> [w245]
        tunnel: w193 -> [w244]
        tunnel: w192 -> [w243]
        tunnel: [w243] -> w191
        tunnel: w184 -> [w242]
        tunnel: w183 -> [w238]
        tunnel: [w238] -> w182
        stop <- w253 stop-if-true
        w240 = u16 0 ("Current Step")
        n309 = Wait on Notification(notifier=w257, ignore previous (F)=TRUE) -> (notifier out=w252:refnum<notifier>, notification=w255:T11)  [unwired: 2 in, 2 out]
        n310 = Unbundle By Name(w255) -> ("Actions"=w250:T12)
        n311 = Bundle By Name(cluster=T21 {"Scan Mode"=enum."Steps Then Cycles", "Current Step"=0, "Current Cycle"=0, "Num of Steps"=0, "Num of Cycles"=0} ("Cycles Steps Tracker"), "Current Step"=w240, "Current Cycle"=w240, "Num of Steps"=w240, "Num of Cycles"=w240, "Scan Mode"="Scan Mode") -> (w247:T21)
        n312 = Equal?(x=w250, y=Orca_Flash_Capture_Actions."Quit") -> (x = y?=w253:bool)
        n313 = while {
          shift-right: [w277] -> _
          shift-left: w250 -> [w258]
          tunnel: w252 -> [w272]
          tunnel: w251 -> [w274]
          tunnel: w250 -> [w273]
          tunnel: w248 -> [w271]
          shift-right: [w269] -> _
          shift-left: w247 -> [w270]
          tunnel: w246 -> [w268]
          tunnel: w245 -> [w267]
          tunnel: w244 -> [w266]
          tunnel: w243 -> [w265]
          tunnel: w242 -> [w264]
          tunnel: w238 -> [w263]
          stop <- w275 stop-if-true
          n314 = case shown="\"Camera\"" w258 {
            selector: w258 -> [_ _ _ _ w410 _ _ _ _ _ _ _ _ _ _ _]
            tunnel: [Orca_Flash_Capture_Actions."Quit" ("y") w282 w303 Orca_Flash_Capture_Actions."Laser Off" ("y") w406 Orca_Flash_Capture_Actions."Start Acquisition" ("y") w486 Orca_Flash_Capture_Actions."Write Metadata" ("y") w615 Orca_Flash_Capture_Actions."Camera" ("y") w646 w716 Orca_Flash_Capture_Actions."Setup" ("y") Orca_Flash_Capture_Actions."External Cycle Sync" ("y") w853 Orca_Flash_Capture_Actions."Quit" ("y")] -> w277
            tunnel: [w279 w301 w306 w369 w408 w436 w488 w564 w623 w642 w683 w742 w757 w819 w874 TRUE] -> w275
            tunnel: FALSE -> [w279 w301 w306 w369 w408 w436 w488 w564 w623 w642 w683 w742 w757 w819 w874 _]
            tunnel: w274 -> [_ w294 _ w366 _ w422 w487 _ _ _ w675 _ _ _ _ _]
            tunnel: w273 -> [_ w289 w302 w365 _ w429 w484 w562 w621 _ _ _ _ _ _ _]
            tunnel: w272 -> [_ _ w304 w363 _ w434 w485 w563 w614 _ w677 w729 w749 w817 _ w906]
            tunnel: w271 -> [_ _ _ w360 _ _ w483 _ _ _ _ _ w748 w818 _ _]
            tunnel: w270 -> [w278 w300 w305 w346 w404 w424 w482 w557 w622 w640 w672 w727 w747 w802 w873 w916]
            tunnel: [w278 w300 w305 w346 w404 w424 w481 w557 w622 w640 w672 w741 w747 w802 w873 w916] -> w269
            tunnel: w268 -> [_ _ _ _ _ w418 _ _ _ _ _ _ _ _ _ _]
            tunnel: w267 -> [_ _ _ _ _ w417 _ _ _ _ _ _ _ _ _ _]
            tunnel: w266 -> [_ _ _ _ _ w416 _ _ _ _ _ _ _ _ _ _]
            tunnel: w265 -> [_ w293 _ _ _ _ w480 _ _ _ w671 _ _ w803 _ w911]
            tunnel: w264 -> [_ _ _ w342 _ _ _ _ _ _ _ _ _ _ _ _]
            tunnel: w263 -> [_ _ _ _ _ _ _ _ _ _ w659 _ _ _ _ _]
            frame "Idle", Default {
            }
            frame "Live Preview", "Capture" {
              w291 = FALSE ("Camera Running?")
              n315 = call "Orca Flash Messanger.vi"("Notifier Name"=w294, "Camera Actions"=Orca_Flash_Actions."STATUS") -> ("Image Ref"=w295:T6)  [unwired: 9 in, 4 out]
              n316 = Equal?(x=w289, y=Orca_Flash_Capture_Actions."Live Preview") -> (x = y?=w281:bool)
              n317 = Select(t="Preview Initiated", s=w281, f="Capture Initiated") -> (s? t:f=w285:string)
              n318 = Get Notifier Status(notifier=w293) -> (notifier out=w298:refnum<notifier>, current notification=w299:T7)  [unwired: 1 in, 3 out]
              n319 = Bundle By Name(cluster=w299, "Image Ref"=w295, "Cycle Number"=u16 0, "Camera Running?"=w291, "Capture?"=w291) -> (w297:T7)
              n320 = call "Log File.vi"("Actions"=Log_File_Actions."Write", "Message"=w285) -> ()  [unwired: 14 in]
              n321 = Send Notification(notification=w297, notifier=w298) -> ()  [unwired: 1 in, 2 out]
              n322 = Select(t=Orca_Flash_Capture_Actions."Laser On" ("y"), s=w281, f=Orca_Flash_Capture_Actions."Check File Name" ("y")) -> (s? t:f=w282:T12)
            }
            frame "Check File Name" {
              n323 = case shown="\"Capture\"" w302 {
                tunnel: w304 -> [_ w319]
                tunnel: [Orca_Flash_Capture_Actions."Laser On" ("y") w311] -> w303
                frame Default {
                }
                frame "Capture" {
                  n324 = Get Notifier Status(notifier=w319) -> (current notification=w318:T11)  [unwired: 1 in, 4 out]
                  n325 = Unbundle By Name(w318) -> ("Base Path"=w313:path)
                  n326 = Strip Path(path=w313) -> (stripped path=w317:path, name=w314:string)
                  n327 = List Folder(path=w317, pattern="*.dcimg") -> (filenames=w315:string[], error out=w310:errorcluster)  [unwired: 2 in, 2 out]
                  n328 = case shown="No Error" w310 {
                    tunnel: w315 -> [w323 _]
                    tunnel: w314 -> [w322 _]
                    tunnel: [w320 FALSE] -> w312
                    frame No Error {
                      n329 = for {
                        tunnel: w323 -> [w331] mode=indexing
                        tunnel: w322 -> [w325]
                        tunnel: [w324] -> w321 mode=indexing
                        n330 = String Length(string=w331) -> (length=w329:i32)
                        n331 = Subtract(x=w329, y=14) -> (x-y=w327:i32)
                        n332 = String Subset(string=w331, offset (0)=0, length (rest)=w327) -> (substring=w326:string)
                        n333 = Equal?(x=w326, y=w325) -> (x = y?=w324:bool)
                      }
                      n334 = Or Array Elements(Boolean array=w321) -> (logical OR=w320:bool)
                    }
                    frame Error {
                      # "If the folder doesn't exist yet, we\nget an error when trying to load\nits contents."
                    }
                  }
                  n335 = case shown="True" w312 {
                    tunnel: [Orca_Flash_Capture_Actions."Laser On" ("y") Orca_Flash_Capture_Actions."Quit" ("y")] -> w311
                    tunnel: ["File name check passed." "Duplicate file name detected. Capture cancelled."] -> w308
                    frame False {
                    }
                    frame True {
                      n336 = local write "Capture"(FALSE ("Capture")) -> ()
                      n337 = One Button Dialog(message="Capture canceled. Change file name and try again.") -> ()  [unwired: 1 in, 1 out]
                    }
                  }
                  n338 = call "Log File.vi"("Actions"=Log_File_Actions."Write", "Message"=w308) -> ()  [unwired: 14 in]
                }
              }
            }
            frame "Abort" {
              w362 = u16 1 ("Current Cycle")
              w367 = FALSE ("Live Preview")
              n339 = call "Orca Flash Messanger.vi"("Notifier Name"=w366, "Camera Actions"=Orca_Flash_Actions."IDLE") -> ()  [unwired: 9 in, 5 out]
              n340 = local write "Live Preview"(w367) -> ()
              n341 = local write "Capture"(w367) -> ()
              n342 = Equal?(x=Orca_Flash_Capture_Actions."Capture", y=w365) -> (x = y?=w359:bool)
              n343 = Get Notifier Status(notifier=w363) -> (current notification=w341:T11)  [unwired: 1 in, 4 out]
              n344 = local write "Current Cycle"(w362) -> ()
              n345 = local write "Current Step"(w362) -> ()
              n346 = Unbundle By Name(w341) -> ("Init Z Position (µm)"=w361:dbl)
              n347 = call "Log File.vi"("Actions"=Log_File_Actions."Write", "Message"="Abort case executed.") -> ()  [unwired: 14 in]
              n348 = Obtain Notifier(name (unnamed)="WFDC External Sync", notification data type=T23 {"Cycle Sync"=enum."Pause Requested", "Z Offset"=0.0, "WFDC Status"=enum."Idle"} ("WFDC External Sync"), create if not found? (T)=FALSE) -> (notifier out=w353:refnum<notifier>, error out=w358:errorcluster)  [unwired: 1 in, 1 out]
              n349 = Get Notifier Status(notifier=w353, error in (no error)=w358) -> (notifier out=w348:refnum<notifier>, current notification=w347:T23, error out=w357:errorcluster)  [unwired: 2 out]
              n350 = Unbundle By Name(w347) -> ("WFDC Status"=w345:T22)
              n351 = Unbundle By Name(w357) -> ("status"=w356:bool)
              n352 = Not Equal?(x=WFDC_Status."DC Active", y=w345) -> (x != y?=w355:bool)
              n353 = Equal?(x=w345, y=WFDC_Status."Error") -> (x = y?=w343:bool)
              n354 = Or(x=w355, y=w356) -> (x .or. y?=w349:bool)
              n355 = case shown="True" w359 {
                tunnel: w361 -> [_ w378]
                tunnel: w360 -> [_ w377]
                tunnel: w349 -> [_ w376]
                tunnel: w348 -> [_ w375]
                tunnel: w347 -> [_ w374]
                tunnel: w343 -> [_ w372]
                tunnel: w342 -> [_ w371]
                frame False {
                }
                frame True {
                  n356 = case shown="True" w376 {
                    tunnel: w378 -> [_ w396]
                    tunnel: w377 -> [_ w395]
                    tunnel: w375 -> [w389 _]
                    tunnel: w374 -> [w388 _]
                    frame False {
                      n357 = Bundle By Name(cluster=w388, "Z Offset"=0.0) -> (w390:T23)
                      n358 = Send Notification(notification=w390, notifier=w389) -> (notifier out=w385:refnum<notifier>)  [unwired: 1 in, 1 out]
                      n359 = Release Notifier(notifier=w385, force destroy? (F)=FALSE) -> ()  [unwired: 1 in, 3 out]
                    }
                    frame True {
                      n360 = Build Array(w396) -> (w391:dbl[])
                      n361 = call "Stages Messenger.vi"("Stage Notifier Name"=w395, "Actions"=Stage_Actions."MOVE", "Setpoint"=w391, "Axis"=bool[] [TRUE], "Exit While Busy?"=FALSE) -> ()  [unwired: 7 in, 4 out]
                    }
                  }
                  n362 = case shown="True" "Email Alerts" {
                    tunnel: w372 -> [_ w381]
                    tunnel: w371 -> [_ w379]
                    frame False {
                    }
                    frame True {
                      n363 = Select(t="Acquisition Error - Abort", s=w381, f="Acquisition Finished") -> (s? t:f=w380:string)
                      n364 = call "SMTP Email Alerts Messenger.vi"("Notifier Name"=w379, "Actions"=SMTP_Email_Alerts_Actions."Send Message", "Subject"=w380, "Body Text"=w380) -> ()  [unwired: 12 in]
                    }
                  }
                }
              }
            }
            frame "Laser On", "Laser Off" {
              n365 = Equal?(x=w410, y=Orca_Flash_Capture_Actions."Laser On") -> (x = y?=w401:bool)
              n366 = Select(t=Laser_Power_Ctrl_Messenger_Actions."All Active On" ("Power Ctrl Actions"), s=w401, f=Laser_Power_Ctrl_Messenger_Actions."All Off" ("Power Ctrl Actions")) -> (s? t:f=w399:T27)
              n367 = call "Laser Power Control Messenger.vi"("Power Ctrl Actions"=w399) -> ()  [unwired: 13 in, 2 out]
              n368 = Select(t=Orca_Flash_Capture_Actions."Set Exposure Time" ("y"), s=w401, f=Orca_Flash_Capture_Actions."Quit" ("y")) -> (s? t:f=w406:T12)
              n369 = Format Into String(initial string="Lasers set to: ", w399) -> (resulting string=w397:string)  [unwired: 2 in, 1 out]
              n370 = call "Log File.vi"("Actions"=Log_File_Actions."Write", "Message"=w397) -> ()  [unwired: 14 in]
            }
            frame "Set Exposure Time" {
              # "Frame Rate (Hz)"
              n371 = Get Notifier Status(notifier=w434) -> (current notification=w430:T11)  [unwired: 1 in, 4 out]
              n372 = Unbundle By Name(w430) -> ("Line Scan?"=w420:bool, "Line Scan Mode"=w419:T3, "Capture Exposure (s)"=w425:dbl, "Preview Exposure (s)"=w426:dbl)
              n373 = Equal?(x=w429, y=Orca_Flash_Capture_Actions."Capture") -> (x = y?=w427:bool)
              n374 = Select(t=w425, s=w427, f=w426) -> (s? t:f=w423:dbl)
              n375 = case shown="False" w420 {
                tunnel: w423 -> [w438 w450]
                tunnel: [w438 w447] -> w415
                tunnel: w422 -> [w441 w449]
                tunnel: [w441 w446] -> w421
                tunnel: w419 -> [_ w445]
                tunnel: w418 -> [w440 w444]
                tunnel: w417 -> [_ w443]
                tunnel: w416 -> [_ w442]
                frame False {
                  # "Exposure Time (s)"
                  n376 = call "AO SCTR Messenger.vi"("Notifier Name"=w440, "Actions"=AO_SCTR_Actions."Stop at Offset", "Offset (V)"=-0.25, "Exposure Time (s)"=w438) -> ()  [unwired: 11 in, 1 out]
                }
                frame True {
                  n377 = To Double Precision Float(number="Number of Lines") -> (double precision float=w448:dbl)
                  n378 = case shown="\"Automatic\"" w445 {
                    tunnel: w450 -> [_ w479]
                    tunnel: w449 -> [w456 w478]
                    tunnel: w448 -> [w454 w477]
                    tunnel: [w452 w476] -> w447
                    tunnel: [w455 w475] -> w446
                    tunnel: w444 -> [_ w469]
                    tunnel: w443 -> [_ w466]
                    tunnel: w442 -> [_ w465]
                    frame Default {
                      n379 = call "Orca Flash Messanger.vi"("Notifier Name"=w456, "Camera Actions"=Orca_Flash_Actions."GETPARAM", "sCMOS Parameter"=T18 {"Value"=0.0, "Parameter"=4226016}) -> ("Notifier Name Dup"=w455:string, "sCMOS Parameter"=w459:T18)  [unwired: 8 in, 3 out]
                      n380 = Unbundle By Name(w459) -> ("Value"=w453:dbl)
                      n381 = Multiply(x=w453, y=w454) -> (x*y=w452:dbl)
                    }
                    frame "Automatic" {
                      n382 = call "Orca Flash Capture Set Interline Interval.vi"("Camera Notifier Name"=w478, "Frame Rate (Hz)"=w479) -> ("Camera Notifier Name (Dup)"=w475:string, "Interline Interval (s)"=w474:dbl)  [unwired: 12 in]
                      n383 = Multiply(x=w474, y=w477) -> (x*y=w476:dbl)
                      n384 = call "Orca Flash Capture Set Auto Waveform.vi"("Interline Interval"=w474, "Filter Index"="Current Filter", "Waveform Parameters"=w466, "Filter Offsets"=w465) -> ("Offset (V)"=w461:dbl, "Amplitude (V)"=w472:dbl, "Samples per Channel"=w471:i32, "Delay (ms)"=w470:dbl, "Line Scan Settings"=w468:T4)  [unwired: 7 in]
                      n385 = local write "Line Scan Settings"(w468) -> ()
                      n386 = Add(x="Line Scan Offset (V)", y=w461) -> (x+y=w463:dbl)
                      n387 = Select(t=w463, s="Line Scan Offset Active", f=w461) -> (s? t:f=w462:dbl)
                      n388 = call "AO SCTR Messenger.vi"("Notifier Name"=w469, "Actions"=AO_SCTR_Actions."Update and Run", "Offset (V)"=w462, "Amplitude (V)"=w472, "Samples Per Channel"=w471, "Start Delay (ms)"=w470) -> ()  [unwired: 9 in, 1 out]
                    }
                  }
                }
              }
              n389 = Format Into String(format string="%04.4f", initial string="Exposure time set to: ", w415) -> (resulting string=w411:string)  [unwired: 1 in, 1 out]
              n390 = Bundle By Name(cluster=T18 {"Value"=0.0, "Parameter"=2049184} ("sCMOS Parameter"), "Value"=w415) -> (w433:T18)
              n391 = call "Log File.vi"("Actions"=Log_File_Actions."Write", "Message"=w411) -> ()  [unwired: 14 in]
              n392 = call "Orca Flash Messanger.vi"("Notifier Name"=w421, "Camera Actions"=Orca_Flash_Actions."SETPARAM", "sCMOS Parameter"=w433) -> ()  [unwired: 8 in, 5 out]
            }
            frame "Start Acquisition" {
              n393 = case shown="\"Capture\"" w484 {
                tunnel: w487 -> [_ w493 _]
                tunnel: [Orca_Flash_Capture_Actions."Quit" ("y") Orca_Flash_Capture_Actions."Quit" ("y") Orca_Flash_Capture_Actions."Update SubFolder" ("y")] -> w486
                tunnel: w485 -> [_ _ w530]
                tunnel: w483 -> [_ _ w522]
                tunnel: w482 -> [w489 w494 w518]
                tunnel: [w489 w494 w517] -> w481
                tunnel: w480 -> [_ _ w510]
                frame Default {
                }
                frame "Live Preview" {
                  n394 = call "Orca Flash Messanger.vi"("Notifier Name"=w493, "Camera Actions"=Orca_Flash_Actions."PREVIEW") -> ()  [unwired: 9 in, 5 out]
                  n395 = call "Log File.vi"("Actions"=Log_File_Actions."Write", "Message"="Live preview started") -> ()  [unwired: 14 in]
                }
                frame "Capture" {
                  w516 = sgl 0.0 ("Cycle")
                  n396 = Get Notifier Status(notifier=w510) -> (notifier out=w514:refnum<notifier>, current notification=w513:T7)  [unwired: 1 in, 3 out]
                  n397 = Bundle By Name(cluster=w513, "Capture?"=TRUE) -> (w512:T7)
                  n398 = call "Stages Messenger.vi"("Stage Notifier Name"=w522, "Actions"=Stage_Actions."Get Position") -> ("Positions"=w525:dbl[])  [unwired: 10 in, 3 out]
                  n399 = Send Notification(notification=w512, notifier=w514) -> ()  [unwired: 1 in, 2 out]
                  n400 = Index Array(array=w525, index=0) -> (element=w523:dbl)
                  n401 = local write "Z Step"(w516) -> ()
                  n402 = local write "Cycle"(w516) -> ()
                  n403 = local write "Frame"(u32 0 ("Frame")) -> ()
                  n404 = Get Notifier Status(notifier=w530) -> (notifier out=w527:refnum<notifier>, current notification=w528:T11)  [unwired: 1 in, 3 out]
                  n405 = Bundle By Name(cluster=w528, "Init Z Position (µm)"=w523) -> (w519:T11)
                  n406 = Unbundle By Name(w519) -> ("Cycles"=w520:u16, "No. of Z Steps"=w521:u16)
                  n407 = Send Notification(notification=w519, notifier=w527) -> ()  [unwired: 1 in, 2 out]
                  n408 = Bundle By Name(cluster=w518, "Num of Cycles"=w520, "Num of Steps"=w521) -> (w517:T21)
                  n409 = Obtain Notifier(name (unnamed)="WFDC External Sync", notification data type=T23 {"Cycle Sync"=enum."Pause Requested", "Z Offset"=0.0, "WFDC Status"=enum."Idle"} ("WFDC External Sync"), create if not found? (T)=FALSE) -> (notifier out=w508:refnum<notifier>, error out=w509:errorcluster)  [unwired: 1 in, 1 out]
                  n410 = call "Log File.vi"("Actions"=Log_File_Actions."Write", "Message"="Start aquisition: capture case") -> ()  [unwired: 14 in]
                  n411 = Get Notifier Status(notifier=w508, error in (no error)=w509) -> (notifier out=w503:refnum<notifier>, current notification=w502:T23, error out=w501:errorcluster)  [unwired: 2 out]
                  n412 = Unbundle By Name(w502) -> ("WFDC Status"=w504:T22)
                  n413 = case shown="\"Error\"" w504 {
                    tunnel: w503 -> [w533 w538]
                    tunnel: w502 -> [_ w537]
                    tunnel: w501 -> [w532 w535]
                    tunnel: [w533 w536] -> w499
                    tunnel: [w532 w534] -> w500
                    frame Default {
                    }
                    frame "Error" {
                      n414 = Two Button Dialog(message="Reset Wide Field Drift Correction error?", 1:"No" ("F button name (\"Cancel\")"), 2:"Yes" ("T button name (\"OK\")")) -> (T button?=w542:bool)
                      n415 = case shown="True" w542 {
                        tunnel: w538 -> [w544 w549]
                        tunnel: w537 -> [_ w551]
                        tunnel: [w544 w547] -> w536
                        tunnel: w535 -> [w543 w546]
                        tunnel: [w543 w545] -> w534
                        frame False {
                        }
                        frame True {
                          n416 = Bundle By Name(cluster=w551, "WFDC Status"=WFDC_Status."Idle") -> (w548:T23)
                          n417 = Send Notification(notification=w548, notifier=w549, error in (no error)=w546) -> (notifier out=w547:refnum<notifier>, error out=w545:errorcluster)
                        }
                      }
                    }
                  }
                  n418 = case shown="No Error" w500 {
                    tunnel: w499 -> [w531 _]
                    frame No Error {
                      n419 = Release Notifier(notifier=w531) -> ()  [unwired: 2 in, 3 out]
                    }
                    frame Error {
                    }
                  }
                }
              }
            }
            frame "Update SubFolder" {
              n420 = Equal?(x=w562, y=Orca_Flash_Capture_Actions."Capture") -> (x = y?=w560:bool)
              n421 = And(x=w560, y="Auto Update Subfolder") -> (x .and. y?=w558:bool)
              n422 = case shown="False" w558 {
                tunnel: w563 -> [w579 w608]
                tunnel: [w566 w589] -> w555
                frame False {
                  w570 = T32 0 items=["both", "start of string", "end of string"] ("location (both)")
                  n423 = Get Notifier Status(notifier=w579) -> (notifier out=w578:refnum<notifier>, current notification=w576:T11)  [unwired: 1 in, 3 out]
                  n424 = Unbundle By Name(w576) -> ("Base Path"=w575:path)
                  n425 = Strip Path(path=w575) -> (stripped path=w574:path, name=w569:string)
                  n426 = call <vilib>:"Check if File or Folder Exists.vi"("path"=w574) -> ("error out"=w571:errorcluster, "file or folder exists?"=w573:bool, "dup path"=w572:path)  [unwired: 8 in]
                  n427 = call <vilib>:"Trim Whitespace.vi"("string"=w569, "location (both)"=w570) -> ("trimmed string"=w567:string)
                  n428 = case shown="False" w573 {
                    tunnel: w572 -> [w582 w583]
                    tunnel: w571 -> [w581 _]
                    tunnel: [w580 w583] -> w568
                    frame False {
                      n429 = Create Folder(path (use dialog)=w582, error in=w581) -> (created path=w580:path)  [unwired: 1 in, 2 out]
                    }
                    frame True {
                    }
                  }
                  n430 = Build Path(base path=w568, name or relative path=w567) -> (appended path=w566:path)
                  n431 = Bundle By Name(cluster=w576, "Save Path"=w566) -> (w577:T11)
                  n432 = Send Notification(notification=w577, notifier=w578) -> ()  [unwired: 1 in, 2 out]
                }
                frame True {
                  w588 = T32 0 items=["both", "start of string", "end of string"] ("location (both)")
                  n433 = Get Notifier Status(notifier=w608) -> (notifier out=w602:refnum<notifier>, current notification=w601:T11)  [unwired: 1 in, 3 out]
                  n434 = Unbundle By Name(w601) -> ("Base Path"=w585:path)
                  n435 = Strip Path(path=w585) -> (stripped path=w584:path, name=w587:string)
                  n436 = feedback #5(u32 0) -> (w603:u32)
                  n437 = feedback-in #6(w584) -> ()
                  n438 = feedback #6(path "") -> (w594:path)
                  n439 = Increment(x=w603) -> (x+1=w591:u32)
                  n440 = Not Equal?(x=w584, y=w594) -> (x != y?=w593:bool)
                  n441 = Select(t=u32 0, s=w593, f=w591) -> (s? t:f=w590:u32)
                  n442 = feedback-in #5(w590) -> ()
                  n443 = Format Into String(format string="%03d", w590) -> (resulting string=w604:string)  [unwired: 2 in, 1 out]
                  n444 = call <vilib>:"Space Constant.vi"() -> ("String"=w596:string)
                  n445 = Concatenate Strings("Subfolder Name", w596, w604) -> (w607:string)
                  n446 = Build Path(base path=w584, name or relative path=w607) -> (appended path=w599:path)
                  n447 = call <vilib>:"Trim Whitespace.vi"("string"=w587, "location (both)"=w588) -> ("trimmed string"=w586:string)
                  n448 = Create Folder(path (use dialog)=w599) -> (created path=w598:path)  [unwired: 2 in, 2 out]
                  n449 = Build Path(base path=w598, name or relative path=w586) -> (appended path=w589:path)
                  n450 = Bundle By Name(cluster=w601, "Save Path"=w589) -> (w600:T11)
                  n451 = Send Notification(notification=w600, notifier=w602) -> ()  [unwired: 1 in, 2 out]
                }
              }
              n452 = Path To String(path=w555) -> (string=w554:string)
              n453 = Concatenate Strings("Save path set to: ", w554) -> (w552:string)
              n454 = call "Log File.vi"("Actions"=Log_File_Actions."Write", "Message"=w552) -> ()  [unwired: 14 in]
            }
            frame "Write Metadata" {
              n455 = Get Notifier Status(notifier=w614) -> (notifier out=w613:refnum<notifier>, current notification=w612:T11)  [unwired: 1 in, 3 out]
              n456 = Unbundle By Name(w612) -> ("Collect Metadata?"=w609:bool)
              n457 = Equal?(x=w621, y=Orca_Flash_Capture_Actions."Capture") -> (x = y?=w611:bool)
              n458 = And(x=w609, y=w611) -> (x .and. y?=w610:bool)
              n459 = case shown="False" w610 {
                tunnel: w613 -> [_ w639]
                tunnel: [errorcluster {"status"=FALSE, "code"=0, "source"=""} ("Write Errror") w631] -> w619
                frame False {
                }
                frame True {
                  n460 = Get Notifier Status(notifier=w639) -> (current notification=w638:T11)  [unwired: 1 in, 4 out]
                  n461 = Unbundle By Name(w638) -> ("Save Path"=w637:path)
                  n462 = call "Write Device Metadata.vi"("File Path"=w637) -> ("File Path (Dup)"=w636:path, "Write Errror"=w635:errorcluster)  [unwired: 13 in]
                  n463 = call "Write Microscope Metadata.vi"("File Path"=w636, "Error In"=w635) -> ("File Path (Dup)"=w633:path, "Write Errror"=w634:errorcluster)  [unwired: 12 in]
                  n464 = call "Run Sample Metadata.vi"("Image File (Path/Name)"=w633, "Error In"=w634) -> ("Error Out"=w631:errorcluster)  [unwired: 12 in, 1 out]
                  n465 = Unbundle By Name(w631) -> ("status"=w630:bool)
                  n466 = Select(t="Error", s=w630, f="No Error") -> (s? t:f=w627:string)
                  n467 = Concatenate Strings("Metadata saved with error status: ", w627) -> (w625:string)
                  n468 = call "Log File.vi"("Actions"=Log_File_Actions."Write", "Message"=w625) -> ()  [unwired: 14 in]
                }
              }
              n469 = Unbundle By Name(w619) -> ("status"=w618:bool)
              n470 = Select(t=Orca_Flash_Capture_Actions."Abort" ("y"), s=w618, f=Orca_Flash_Capture_Actions."Setup" ("y")) -> (s? t:f=w615:T12)
            }
            frame "Setup" {
              # "Change lasers here"
            }
            frame "Camera" {
              n471 = Get Notifier Status(notifier=w677) -> (notifier out=w682:refnum<notifier>, current notification=w673:T11)  [unwired: 1 in, 3 out]
              n472 = Unbundle By Name(w672) -> ("Current Cycle"=w650:u16, "Current Step"=w676:u16)
              n473 = Unbundle By Name(w673) -> ("Save Path"=w679:path, "Frames"=w674:u32)
              n474 = call "Orca Flash Capture File Name Increment.vi"("Path In"=w679, "Cycle"=w650, "Step"=w676) -> ("Path Out"=w660:path)  [unwired: 12 in]
              n475 = Format Into String(format string="%03d", initial string="Cycle: ", w650) -> (resulting string=w647:string)  [unwired: 1 in, 1 out]
              n476 = call "Log File.vi"("Actions"=Log_File_Actions."Write", "Message"=w647) -> ()  [unwired: 14 in]
              n477 = call "Orca Flash Messanger.vi"("Notifier Name"=w675, "Camera Actions"=Orca_Flash_Actions."Record Settings", "Path"=w660, "# of frames"=w674) -> ("Notifier Name Dup"=w681:string)  [unwired: 7 in, 4 out]
              n478 = call "Orca Flash Messanger.vi"("Notifier Name"=w681, "Camera Actions"=Orca_Flash_Actions."RECORD") -> ("Notifier Name Dup"=w656:string, "Image Ref"=w657:T6)  [unwired: 9 in, 3 out]
              n479 = Get Notifier Status(notifier=w671) -> (notifier out=w670:refnum<notifier>, current notification=w669:T7)  [unwired: 1 in, 3 out]
              n480 = Bundle By Name(cluster=w669, "Camera Running?"=TRUE) -> (w667:T7)
              n481 = while {
                tunnel: w656 -> [w688]
                tunnel: [w685] -> w655
                tunnel: ["Camera record started" ("Message")] -> w653
                stop <- w687 stop-if-true
                n482 = call "Orca Flash Messanger.vi"("Notifier Name"=w688, "Camera Actions"=Orca_Flash_Actions."STATUS") -> ("Notifier Name Dup"=w685:string, "Running?"=w687:bool)  [unwired: 9 in, 3 out]
                n483 = Wait (ms)(milliseconds to wait=u32 2) -> ()  [unwired: 1 out]
              }
              n484 = call "Log File.vi"("Actions"=Log_File_Actions."Write", "Message"=w653) -> ()  [unwired: 14 in]
              n485 = Send Notification(notification=w667, notifier=w670) -> (notifier out=w666:refnum<notifier>)  [unwired: 1 in, 1 out]
              n486 = while {
                tunnel: w655 -> [w712]
                tunnel: [w709] -> w646
                tunnel: w682 -> [w699]
                tunnel: w657 -> [w698]
                tunnel: [w692] -> w662
                tunnel: w666 -> [w692]
                tunnel: w660 -> [w691]
                tunnel: [w691] -> w658
                stop <- w705 stop-if-true
                n487 = Get Notifier Status(notifier=w699) -> (current notification=w711:T11)  [unwired: 1 in, 4 out]
                n488 = Unbundle By Name(w711) -> ("Running?"=w690:bool)
                n489 = Wait (ms)(milliseconds to wait=u32 25) -> ()  [unwired: 1 out]
                n490 = call "IMAQ Read Custom Data"("Key"="Image Data", "Image"=w698) -> ("Custom Data Out"=w696:string)  [unwired: 7 in, 2 out]
                n491 = Unflatten From JSON(JSON string=w696, type and defaults=T29 {"Frame"=0, "Sensor Height"=0, "Sensor Width"=0, "ROI Height"=0, "ROI Width"=0, "ROI Enable?"=FALSE, "Bit per Pixel"=0} ("Camera IMAQ Key Info")) -> (value=w694:T29)  [unwired: 5 in, 1 out]
                n492 = Not(x=w690) -> (.not. x?=w708:bool)
                n493 = Unbundle By Name(w694) -> ("Frame"=→"Frame" →"Current Frame":u32)
                n494 = Select(t=Orca_Flash_Actions."STATUS" ("Camera Actions"), s=w690, f=Orca_Flash_Actions."IDLE") -> (s? t:f=w700:T20)
                n495 = call "Orca Flash Messanger.vi"("Notifier Name"=w712, "Camera Actions"=w700) -> ("Running?"=w707:bool)  [unwired: 9 in, 4 out]
                n496 = Not(x=w707) -> (.not. x?=w706:bool)
                n497 = Or(x=w708, y=w706) -> (x .or. y?=w705:bool)
                n498 = Select(t=Orca_Flash_Capture_Actions."Switch" ("y"), s=w690, f=Orca_Flash_Capture_Actions."Abort") -> (s? t:f=w709:T12)
              }
              n499 = Get Notifier Status(notifier=w662) -> (notifier out=w661:refnum<notifier>, current notification=w663:T7)  [unwired: 1 in, 3 out]
              n500 = Bundle By Name(cluster=w663, "Camera Running?"=FALSE) -> (w665:T7)
              n501 = Format Into String(initial string="Camera stopped status: ", w646) -> (resulting string=w644:string)  [unwired: 2 in, 1 out]
              n502 = call "Log File.vi"("Actions"=Log_File_Actions."Write", "Message"=w644) -> ()  [unwired: 14 in]
              n503 = Send Notification(notification=w665, notifier=w661) -> ()  [unwired: 1 in, 2 out]
              n504 = Enqueue Element(queue=w659, element=w658, timeout in ms (-1)=30000) -> ()  [unwired: 1 in, 3 out]
            }
            frame "Switch" {
              n505 = Get Notifier Status(notifier=w729) -> (current notification=w728:T11)  [unwired: 1 in, 4 out]
              n506 = Unbundle By Name(w728) -> ("Cycles"=w724:u16, "No. of Z Steps"=w725:u16)
              n507 = Bundle By Name(cluster=w727, "Num of Cycles"=w724, "Num of Steps"=w725) -> (w726:T21)
              n508 = Unbundle By Name(w726) -> ("Current Cycle"=w738:u16, "Num of Cycles"=w737:u16, "Current Step"=w736:u16, "Num of Steps"=w735:u16)
              n509 = Increment(x=w738) -> (x+1=w722:u16)
              n510 = Increment(x=w736) -> (x+1=w721:u16)
              n511 = To Single Precision Float(number=w722) -> (single precision float=w734:sgl)
              n512 = To Single Precision Float(number=w737) -> (single precision float=w733:sgl)
              n513 = To Single Precision Float(number=w721) -> (single precision float=w732:sgl)
              n514 = To Single Precision Float(number=w735) -> (single precision float=w731:sgl)
              n515 = Divide(x=w734, y=w733) -> (x/y=→"Cycle":sgl)
              n516 = Divide(x=w732, y=w731) -> (x/y=→"Z Step":sgl)
              n517 = call "Orca Flash Capture Scan Counter Cycles Steps.vi"("Cycles Steps Tracker"=w726) -> ("Cycles Steps Tracker Out"=w741:T21, "Change Cycle?"=w719:bool, "Done?"=w740:bool)  [unwired: 8 in]
              n518 = Select(t=Orca_Flash_Capture_Actions."Cycle" ("y"), s=w719, f=Orca_Flash_Capture_Actions."Step") -> (s? t:f=w717:T12)
              n519 = Select(t=Orca_Flash_Capture_Actions."Abort" ("y"), s=w740, f=w717) -> (s? t:f=w716:T12)
              n520 = case shown="\"Cycle\"" w716 {
                tunnel: w722 -> [_ w744 _]
                tunnel: w721 -> [_ _ w746]
                frame Default {
                }
                frame "Cycle" {
                  n521 = Increment(x=w744) -> (x+1=→"Current Cycle":u16)
                }
                frame "Step" {
                  n522 = Increment(x=w746) -> (x+1=→"Current Step":u16)
                }
              }
              n523 = Format Into String(initial string="Switch status: ", w716) -> (resulting string=w713:string)  [unwired: 2 in, 1 out]
              n524 = call "Log File.vi"("Actions"=Log_File_Actions."Write", "Message"=w713) -> ()  [unwired: 14 in]
            }
            frame "Step" {
              n525 = Get Notifier Status(notifier=w749) -> (current notification=w750:T11)  [unwired: 1 in, 4 out]
              n526 = Unbundle By Name(w750) -> ("Z Step Size (µm)"=w756:dbl, "No. of Z Steps"=w753:u16)
              n527 = Less?(x=w753, y=u16 2) -> (x < y?=w754:bool)
              n528 = Equal To 0?(x=w756) -> (x = 0?=w751:bool)
              n529 = Or(x=w751, y=w754) -> (x .or. y?=w752:bool)
              n530 = case shown="False" w752 {
                tunnel: w748 -> [w778 _]
                tunnel: w756 -> [w760 _]
                tunnel: w747 -> [w765 _]
                frame False {
                  n531 = Unbundle By Name(w765) -> ("Current Step"=w764:u16)
                  n532 = Obtain Notifier(name (unnamed)="WFDC External Sync", notification data type=T23 {"Cycle Sync"=enum."Pause Requested", "Z Offset"=0.0, "WFDC Status"=enum."Idle"} ("WFDC External Sync"), create if not found? (T)=FALSE) -> (notifier out=w771:refnum<notifier>, error out=w777:errorcluster)  [unwired: 1 in, 1 out]
                  n533 = Get Notifier Status(notifier=w771, error in (no error)=w777) -> (notifier out=w766:refnum<notifier>, current notification=w763:T23, error out=w776:errorcluster)  [unwired: 2 out]
                  n534 = Unbundle By Name(w763) -> ("WFDC Status"=w772:T22)
                  n535 = Unbundle By Name(w776) -> ("status"=w775:bool)
                  n536 = Not Equal?(x=WFDC_Status."DC Active", y=w772) -> (x != y?=w774:bool)
                  n537 = Or(x=w774, y=w775) -> (x .or. y?=w767:bool)
                  n538 = case shown="True" w767 {
                    tunnel: w778 -> [_ w796]
                    tunnel: w760 -> [w786 w795]
                    tunnel: w766 -> [w783 _]
                    tunnel: w764 -> [w788 _]
                    tunnel: w763 -> [w787 _]
                    tunnel: [u32 350 ("milliseconds to wait") u32 100 ("milliseconds to wait")] -> w762
                    tunnel: ["WFDC Z step" "Piezo stage Z step"] -> w759
                    frame False {
                      n539 = To Double Precision Float(number=w788) -> (double precision float=w785:dbl)
                      n540 = Multiply(x=w786, y=w785) -> (x*y=w784:dbl)
                      n541 = Bundle By Name(cluster=w787, "Z Offset"=w784) -> (w782:T23)
                      n542 = Send Notification(notification=w782, notifier=w783) -> (notifier out=w780:refnum<notifier>)  [unwired: 1 in, 1 out]
                      n543 = Release Notifier(notifier=w780) -> ()  [unwired: 2 in, 3 out]
                    }
                    frame True {
                      n544 = Build Array(w795) -> (w794:dbl[])
                      n545 = call "Stages Messenger.vi"("Stage Notifier Name"=w796, "Actions"=Stage_Actions."MVR", "Setpoint"=w794, "Axis"=bool[] [TRUE], "Exit While Busy?"=FALSE) -> ()  [unwired: 7 in, 4 out]
                    }
                  }
                  n546 = Wait (ms)(milliseconds to wait=w762) -> ()  [unwired: 1 out]
                  n547 = call "Log File.vi"("Actions"=Log_File_Actions."Write", "Message"=w759) -> ()  [unwired: 14 in]
                }
                frame True {
                }
              }
            }
            frame "Cycle" {
              n548 = Unbundle By Name(w802) -> ("Scan Mode"=w801:T2, "Current Cycle"=w804:u16)
              n549 = Equal?(x=Orca_Flash_Switch_Cycles_Steps."Cycles Then Steps", y=w801) -> (x = y?=w799:bool)
              n550 = Get Notifier Status(notifier=w817) -> (current notification=w816:T11)  [unwired: 1 in, 4 out]
              n551 = Get Notifier Status(notifier=w803) -> (notifier out=w807:refnum<notifier>, current notification=w806:T7)  [unwired: 1 in, 3 out]
              n552 = Bundle By Name(cluster=w806, "Cycle Number"=w804) -> (w805:T7)
              n553 = Unbundle By Name(w816) -> ("Init Z Position (µm)"=w808:dbl, "Z Step Size (µm)"=w812:dbl, "No. of Z Steps"=w811:u16)
              n554 = Send Notification(notification=w805, notifier=w807) -> ()  [unwired: 1 in, 2 out]
              n555 = Equal To 0?(x=w812) -> (x = 0?=w815:bool)
              n556 = Less?(x=w811, y=u16 2) -> (x < y?=w814:bool)
              n557 = Compound Arithmetic op=OR(w815, w814, w799) -> (w810:bool)
              n558 = case shown="False" w810 {
                tunnel: w818 -> [w822 _]
                tunnel: w808 -> [w824 _]
                tunnel: ["Return to initial Z position done" ("name (unnamed)") "Cycle case executed" ("Message")] -> w797
                frame False {
                  n559 = Obtain Notifier(name (unnamed)="WFDC External Sync", notification data type=T23 {"Cycle Sync"=enum."Pause Requested", "Z Offset"=0.0, "WFDC Status"=enum."Idle"} ("WFDC External Sync"), create if not found? (T)=FALSE) -> (notifier out=w830:refnum<notifier>, error out=w836:errorcluster)  [unwired: 1 in, 1 out]
                  n560 = Get Notifier Status(notifier=w830, error in (no error)=w836) -> (notifier out=w825:refnum<notifier>, current notification=w823:T23, error out=w835:errorcluster)  [unwired: 2 out]
                  n561 = Unbundle By Name(w823) -> ("WFDC Status"=w831:T22)
                  n562 = Unbundle By Name(w835) -> ("status"=w834:bool)
                  n563 = Not Equal?(x=WFDC_Status."DC Active", y=w831) -> (x != y?=w833:bool)
                  n564 = Or(x=w833, y=w834) -> (x .or. y?=w826:bool)
                  n565 = case shown="False" w826 {
                    tunnel: w825 -> [w840 _]
                    tunnel: w824 -> [_ w845]
                    tunnel: w823 -> [w839 _]
                    tunnel: w822 -> [_ w844]
                    tunnel: [u32 350 ("milliseconds to wait") u32 100 ("milliseconds to wait")] -> w821
                    frame False {
                      n566 = Bundle By Name(cluster=w839, "Z Offset"=0.0) -> (w842:T23)
                      n567 = Send Notification(notification=w842, notifier=w840) -> (notifier out=w841:refnum<notifier>)  [unwired: 1 in, 1 out]
                      n568 = Release Notifier(notifier=w841) -> ()  [unwired: 2 in, 3 out]
                    }
                    frame True {
                      n569 = Build Array(w845) -> (w846:dbl[])
                      n570 = call "Stages Messenger.vi"("Stage Notifier Name"=w844, "Actions"=Stage_Actions."MOVE", "Setpoint"=w846, "Axis"=bool[] [TRUE], "Exit While Busy?"=FALSE) -> ()  [unwired: 7 in, 4 out]
                    }
                  }
                  n571 = Wait (ms)(milliseconds to wait=w821) -> ()  [unwired: 1 out]
                }
                frame True {
                }
              }
              n572 = call "Log File.vi"("Actions"=Log_File_Actions."Write", "Message"=w797) -> ()  [unwired: 14 in]
            }
            frame "External Cycle Sync" {
              n573 = Obtain Notifier(name (unnamed)="WFDC External Sync", notification data type=T23 {"Cycle Sync"=enum."Pause Requested", "Z Offset"=0.0, "WFDC Status"=enum."Idle"} ("WFDC External Sync"), create if not found? (T)=FALSE) -> (notifier out=w869:refnum<notifier>, error out=w872:errorcluster)  [unwired: 1 in, 1 out]
              n574 = Get Notifier Status(notifier=w869, error in (no error)=w872) -> (notifier out=w858:refnum<notifier>, current notification=w857:T23, error out=w871:errorcluster)  [unwired: 2 out]
              n575 = Unbundle By Name(w871) -> ("status"=w865:bool)
              n576 = Unbundle By Name(w857) -> ("WFDC Status"=w856:T22, "Cycle Sync"=w864:T24)
              n577 = Not(x=w865) -> (.not. x?=w860:bool)
              n578 = Equal?(x=WFDC_Status."Error", y=w856) -> (x = y?=w852:bool)
              n579 = Equal?(x=WFDC_Status."DC Active", y=w856) -> (x = y?=w862:bool)
              n580 = Equal?(x=w864, y=WFDC_Cycle_Pause."Pause Requested") -> (x = y?=w861:bool)
              n581 = Compound Arithmetic op=AND(w862, w861, w860) -> (w859:bool)
              n582 = case shown="False" w859 {
                tunnel: w858 -> [_ w891]
                tunnel: w857 -> [_ w892]
                frame False {
                  n583 = call "Log File.vi"("Actions"=Log_File_Actions."Write", "Message"="No Ext Syc request") -> ()  [unwired: 14 in]
                }
                frame True {
                  w881 = WFDC_Cycle_Pause."Resumed" ("Cycle Sync")
                  w884 = WFDC_Cycle_Pause."Paused" ("Cycle Sync")
                  n584 = Bundle By Name(cluster=w892, "Cycle Sync"=w884) -> (w890:T23)
                  n585 = Format Into String(initial string="Ext Syc: ", w884) -> (resulting string=w877:string)  [unwired: 2 in, 1 out]
                  n586 = call "Log File.vi"("Actions"=Log_File_Actions."Write", "Message"=w877) -> ()  [unwired: 14 in]
                  n587 = Send Notification(notification=w890, notifier=w891) -> (notifier out=w889:refnum<notifier>)  [unwired: 1 in, 1 out]
                  n588 = while {
                    tunnel: w889 -> [w903]
                    tunnel: [w894] -> w887
                    tunnel: [w893] -> w888
                    i -> [w899]
                    stop <- w895 stop-if-true
                    n589 = Get Notifier Status(notifier=w903) -> (notifier out=w894:refnum<notifier>, current notification=w893:T23)  [unwired: 1 in, 3 out]
                    n590 = Greater?(x=w899, y=180000) -> (0:w896:bool)
                    n591 = Unbundle By Name(w893) -> ("Cycle Sync"=w902:T24)
                    n592 = Equal?(x=w902, y=WFDC_Cycle_Pause."Resume Requested") -> (x = y?=w897:bool)
                    n593 = Or(x=w897, y=w896) -> (x .or. y?=w895:bool)
                    n594 = Wait (ms)(milliseconds to wait=u32 1) -> ()  [unwired: 1 out]
                  }
                  n595 = Bundle By Name(cluster=w888, "Cycle Sync"=w881) -> (w886:T23)
                  n596 = Format Into String(initial string="Ext Syc: ", w881) -> (resulting string=w879:string)  [unwired: 2 in, 1 out]
                  n597 = Send Notification(notification=w886, notifier=w887) -> (notifier out=w885:refnum<notifier>)  [unwired: 1 in, 1 out]
                  n598 = Release Notifier(notifier=w885) -> ()  [unwired: 2 in, 3 out]
                  n599 = call "Log File.vi"("Actions"=Log_File_Actions."Write", "Message"=w879) -> ()  [unwired: 14 in]
                }
              }
              n600 = Select(t=Orca_Flash_Capture_Actions."Abort" ("y"), s=w852, f=Orca_Flash_Capture_Actions."Setup" ("y")) -> (s? t:f=w853:T12)
            }
            frame "Quit" {
              w915 = FALSE ("Capture?")
              n601 = Get Notifier Status(notifier=w906) -> (notifier out=w910:refnum<notifier>, current notification=w909:T11)  [unwired: 1 in, 3 out]
              n602 = Bundle By Name(cluster=w909, "Running?"=FALSE) -> (w907:T11)
              n603 = Send Notification(notification=w907, notifier=w910) -> ()  [unwired: 1 in, 2 out]
              n604 = Get Notifier Status(notifier=w911) -> (notifier out=w914:refnum<notifier>, current notification=w913:T7)  [unwired: 1 in, 3 out]
              n605 = Bundle By Name(cluster=w913, "Camera Running?"=w915, "Capture?"=w915) -> (w912:T7)
              n606 = Send Notification(notification=w912, notifier=w914) -> ()  [unwired: 1 in, 2 out]
              n607 = call "Log File.vi"("Actions"=Log_File_Actions."Write", "Message"="Quit case executed") -> ()  [unwired: 14 in]
            }
          }
          n608 = Format Into String(w258) -> (resulting string=w259:string)  [unwired: 3 in, 1 out]
          n609 = Concatenate Strings("Loop Action: ", w259) -> (w260:string)
          n610 = call "Log File.vi"("Actions"=Log_File_Actions."Write", "Message"=w260) -> ()  [unwired: 14 in]
        }
      }
      n611 = local write "Quit"(w231) -> ()
      n612 = Release Notifier(notifier=w191) -> ()  [unwired: 2 in, 3 out]
      n613 = Release Queue(queue=w182) -> ()  [unwired: 2 in, 3 out]
    }
    frame Error {
      n614 = Release Notifier(notifier=w1316) -> (error out=w1315:errorcluster)  [unwired: 2 in, 2 out]
      n615 = for {
        tunnel: w1314 -> [w1321] mode=indexing
        n616 = call "IMAQ Dispose"("Image"=w1321) -> ()  [unwired: 5 in, 1 out]
      }
      n617 = Unbundle By Name(w1315) -> ("source"=w1318:string)
      n618 = Concatenate Strings("Orca Flash capture manager could not start.", "\r", w1318) -> (w1317:string)
      n619 = One Button Dialog(message=w1317) -> ()  [unwired: 1 in, 1 out]
    }
  }
  n620 = control-ref of="This VI"() -> (w118:refnum<vi>)
  n621 = property class="VI"(reference=w118) -> (reference out=w127:refnum<vi>, "Panel"=w119:refnum<vi>)  [unwired: 1 in, 1 out]
  n622 = property class="Pnl"(reference=w119) -> ("Decos[]"=w117:refnum<vi>[], "Panes[]"=w123:refnum<vi>[])  [unwired: 1 in, 2 out]
  n623 = Array Size(array=w117) -> (size(s)=w115:i32)
  n624 = Decrement(x=w115) -> (x-1=w116:i32)
  n625 = Index Array(array=w123, index=0) -> (element=w122:refnum<vi>)
  n626 = Index Array(array=w117, index=w116) -> (element=w125:refnum<vi>)
  n627 = property class="VI"(reference=w127) -> (reference out=w129:refnum<vi>, "Front Panel.PanelBounds"=w130:T33)  [unwired: 1 in, 1 out]
  n628 = property class="Decor"(reference=w125) -> ("Bounds"=w128:T34)  [unwired: 1 in, 2 out]
  n629 = property class="Pane"(reference=w122, "Origin"=T14 {"Horizontal"=0, "Vertical"=0}, "HorizScrollbarVisibility"=w126, "VertScrollbarVisibility"=w126) -> ()  [unwired: 1 in, 2 out]
  n630 = Unbundle By Name(w128) -> ("Width"=w133:u32, "Height"=w136:u32)
  n631 = control-ref of="Quit"() -> (w120:refnum<vi>)
  n632 = To Word Integer(number=w133) -> (16bit integer=w135:i16)
  n633 = To Word Integer(number=w136) -> ()  [unwired: 1 out]
  n634 = property class="Bool (strict)"(reference=w120) -> ("Height"=w138:u32, "Top"=w139:i32)  [unwired: 1 in, 2 out]
  n635 = Unbundle By Name(w130) -> ("Left"=w132:i16, "Top"=w143:i16)
  n636 = To Word Integer(number=w138) -> (16bit integer=w141:i16)
  n637 = To Word Integer(number=w139) -> (16bit integer=w142:i16)
  n638 = Add(x=w132, y=w135) -> (x+y=w134:i16)
  n639 = Compound Arithmetic op=ADD(w143, w141, w142, i16 12 ("y")) -> (w137:i16)
  n640 = Bundle By Name(cluster=w130, "Right"=w134, "Bottom"=w137) -> (w131:T33)
  n641 = property class="VI"(reference=w129, "Front Panel.PanelBounds"=w131) -> ()  [unwired: 1 in, 2 out]
